vi "GUI_Bella_Control_Center.vi"() -> ()   [LabVIEW 2020]
uses:
  Shared/GUI_Template/GUI_master/tcp_new_data_event.ctl
  Shared/GUI_Template/GUI_master/tcp new data cluster.ctl
  GUI_TestStand/Fire button.ctl
  Device Drivers/DG645/subVIs/TriggerSource_TypDef.ctl
  <vilib>/Utility/config.llb/Write Key (I32).vi
  <vilib>/Platform/browser.llb/Open URL in Default Browser (string).vi
  <vilib>/Utility/config.llb/NI_LVConfig.lvlib
  <vilib>/Utility/config.llb/Read Key (Double).vi
  <vilib>/Utility/config.llb/Write Key (Double).vi
panel:
  in  "delay.Channel_D::32":dbl caption="jet open time D" min=-0.1 max=0.1 format="%.3p"
  in  "delay.Channel_C::32":dbl caption="jet open C" min=-0.1 max=0.1 format="%.3p"
  out "CurrentStatus":string
  in  "MoveStage":bool
  in  "Position.Ch1::44":dbl caption="Current Position" min=0.0 max=150.0
  in  "GUIdevice 44":string="STAGE-LT-Megattenuator"
  in  "GUIdevice 43":string="MANPAR-BELLA-OFI-Boolean"
  in  "GUIdevice 42":string="MANPAR-BELLA-OFI"
  in  "Pressure.device 2::39":dbl caption="Backing pressure" min=-20.0 max=500.0 format="%.3f"
  in  "read config":bool caption="LogTable"
  in  "value5::42":dbl=566.0 caption="2BL probe 0 time pos" min=-9999999.0 max=9999999.0 format="%#_13g"
  in  "save config":bool caption="LogTable"
  in  "configuration file path":path=path "N:/Software/GEECS/user data/BCC.ini"
  out "HPD2 to match HPD":dbl
  in  "Save screenshots":bool
  out "error out":errorcluster
  out "Hpd pos for jet exit":dbl
  in  "value2::42":dbl=276.0 caption="jet exit on hpd for hexX=0" min=-9999999.0 max=9999999.0
  in  "GUIdevice 41":string="STAGE-PL1-JetLength"
  in  "position::41":dbl caption="Jet Length pos" min=0.0 max=50.0 format="%.1f"
  out "lp mode HPDplane\n - HPD ref pos":dbl
  out "height above jet":dbl
  in  "value3::42":dbl=2.6 caption="zpos for 0 above jet" min=-9999999.0 max=9999999.0
  out "HPD - focus":dbl
  in  "value1::42":dbl=230.0 caption="focus on HPD" min=-9999999.0 max=9999999.0
  out "1BL wrt 2BL probe":dbl
  out "1BL delay (ns)\n+ is 1BL after 2BL":dbl
  out "probe delay (ns)\n+ is probe after":dbl caption="probe delay (ns)\n+ is probe after 2BL"
  in  "position::40":dbl caption="2BL probe delay (mm)" min=0.0 max=578.0 format="%.1f"
  in  "GUIdevice 40":string="STAGE-2BL-ProbeDelay"
  in  "Position.Axis 1::8":dbl caption="1BL delay (mm)" min=-500.0 max=500.0 format="%.1f"
  in  "GUIdevice 8":string="STAGE-LT-1BLDelay"
  in  "value4::42":dbl=0.006 caption="JetOnTime" min=-9999999.0 max=9999999.0 format="%#_6p"
  in  "Position.Channel 5::25":dbl caption="SMFiber (1in, 45out)" min=-60.0 max=55.0 format="%.1f"
  in  "value1::43":bool=TRUE caption="GasJetOn"
  in  "value0::43":bool=TRUE caption="ShotControl"
  in  "Thales.DIAG_CU_Output_Percent_1::37":dbl caption="Amp2 att (%)" min=1.0 max=100.0 step=500.0 format="%.2f"
  in  "GUIdevice 37":string="SVE-LT-Thales"
  in  "Pressure.device 1::39":dbl caption="Backing pressure" min=-20.0 max=500.0 format="%.3f"
  in  "GUIdevice 39":string="PRC-PL1-HighPressure"
  in  "Scan":T1(ring)
  in  "LogTable":bool
  in  "New Google\nExpLog for new day?":bool=TRUE
  out "standard output":string
  in  "Create Log":bool caption="LogTable"
  in  "GUIdevice 38":string="STAGE-2BL-Compressor"
  in  "Position.Axis 1::38":dbl caption="Comp2 Translation" min=0.0 max=20.0 format="%.3f"
  in  "Position.Channel 5::31":T2(ring) caption="FROG foil"
  in  "Position.Channel 2::31":T2(ring) caption="Little Rick"
  in  "AnalogOutput.Channel 1::36":dbl caption="M4A att (V)" min=0.0 max=5.0 step=500.0 format="%.2f"
  in  "GUIdevice 36":string="ATT-2BL-M4A"
  in  "GUIdevice 35":string="ATT-2BL-DM"
  in  "AnalogOutput.Channel 1::35":dbl caption="2BL DM att (V)" min=0.0 max=5.0 step=500.0 format="%.2f"
  in  "Step size 2":dbl=20.0 caption="Step size" min=-22.0 max=22.0
  in  "Position.Axis 4::33":dbl caption="Holy M V F4" min=-100000.0 max=100000.0 step=500.0
  in  "Position.Axis 3::33":dbl caption="Holy M H F3" min=-1000000.0 max=1000000.0 step=500.0
  in  "Position.Axis 2::33":dbl caption="Bessel M3 V F2" min=-100000.0 max=100000.0 step=500.0
  in  "Position.Axis 1::33":dbl caption="Bessel M3 H F1" min=-100000.0 max=100000.0 step=500.0
  in  "GUIdevice 33":string="MCD-PL1-picosOFI1"
  in  "delay.Channel_B::32":dbl caption="jet open time B" min=-0.1 max=0.1 format="%.3p"
  in  "delay.Channel_A::32":dbl caption="jet open A" min=-0.1 max=0.1 format="%.3p"
  in  "GUIdevice 32":string="DDG-AA-SRSGasJet-645"
  in  "position::6":dbl caption="LPmode stage long (605 safe)" min=0.0 max=605.0 format="%.1f"
  in  "GUIdevice 6":string="STAGE-PL1-LPmodeLong"
  in  "EnableMotor::6":bool caption="LPmode motor \nstatus"
  in  "position::4":dbl=-1.631e-06 caption="Capstage" min=0.0 max=600.0 format="%.1f"
  in  "GUIdevice 4":string="STAGE-PL1-Capstage1"
  in  "GUIdevice 31":string="1WIRE-BELLA-Flipper"
  in  "Amplitude.Ch GH::10":dbl=-1.631e-06 caption="Shot Shutter V" min=0.5 max=5.0 format="%.1f"
  in  "Rate (Hz)":dbl=0.3
  out "Crystal2":enum16{"In", "Out", "Unknown"}(ring)
  out "Hex1posdesc":enum16{"guiding", "fiber ref", "Unknown"}(ring) caption="Hex1"
  in  "GUIdevice 29":string="MCD-HEAT-ESP0"
  in  "Position.Axis 2::29":dbl caption="Y" min=-5.0 max=25.0 format="%.4f"
  in  "Position.Axis 1::29":dbl caption="X" min=-5.0 max=25.0 format="%.4f"
  in  "wangle::28":dbl caption="w" min=-2.0 max=2.0 step=0.01 format="%.5f"
  in  "vangle::28":dbl caption="v" min=-5.0 max=5.0 step=0.01 format="%.5f"
  in  "uangle::28":dbl caption="u" min=-1.0 max=1.0 step=0.01 format="%.5f"
  in  "ypos::28":dbl caption="y" min=-3.0 max=3.0 step=0.01 format="%.5f"
  in  "zpos::28":dbl caption="z" min=-12.5 max=12.5 step=0.01 format="%.5f"
  in  "xpos::28":dbl caption="x" min=-0.5 max=0.5 step=0.01 format="%.5f"
  in  "GUIdevice 28":string="HEX-PL1-2"
  in  "delay.Channel_A::27":dbl caption="Disch timing both caps" min=-0.1 max=0.1 format="%.3p"
  out "Boolean":bool
  in  "amplitude.Channel_A::27":dbl caption="Caps Trig (V)" min=-3.0 max=4.0 format="%.2f"
  in  "GUIdevice 27":string="DDG-AA-SRS3"
  in  "GUIdevice 26":string="PRC-PL1-PressureAPL"
  in  "pressure::26":dbl caption="Cap2 Pressure (Torr)" min=0.0 max=50.0 format="%.2f"
  in  "Position.Channel 5::25":dbl caption="Wedge (43.5,2)" min=-60.0 max=55.0 format="%.1f"
  in  "Position.Channel 4::25":dbl caption="ND2 (4,45)" min=-35.0 max=-12.0 format="%.1f"
  in  "Position.Channel 1::25":dbl caption="LPmode kicker (~1in, 75out)" min=-75.0 max=79.0 format="%.1f"
  in  "Position.Channel 1::25":dbl caption="ND3 (4,45)" min=-75.0 max=79.0 format="%.1f"
  out "Data.Channel 2::14":dbl caption="Flow US (sccm)" min=0.0 max=1000.0 format="%.1f"
  out "pressure2::5":dbl caption="PDR US (Torr)" min=-100.0 max=500.0 format="%.2f"
  in  "Data.Channel 2::11":dbl caption="Pressure US (Torr)" min=0.0 max=1000.0 format="%.2f"
  in  "GUIdevice 25":string="STAGE-PL1-Smaract"
  in  "Heater Alignment Directions":bool
  in  "Position.Axis 3::15":dbl caption="XY" min=-3.0 max=16.0 format="%.4f"
  in  "Position.Axis 2::15":dbl caption="Y" min=-3.0 max=17.0 format="%.4f"
  in  "Position.Axis 1::15":dbl caption="X" min=-3.0 max=13.0 format="%.4f"
  in  "GUIdevice 24":string="STAGE-HEAT-TL1"
  in  "Encoder position::23":dbl caption="position HPD2" min=0.0 max=600.0 format="%.1f"
  in  "position::3":dbl caption="position HPD" min=0.0 max=600.0 format="%.1f"
  in  "GUIdevice 23":string="STAGE-HPD-Far"
  in  "GUIdevice 22":string="MANPAR-BELLA-FireCont"
  in  "Allow Fire Continues":bool
  out "Fire continues Indicator":bool caption="firing"
  in  "Fire Button":T3=TRUE
  in  "Trigger.Source::10":T4 caption="SRS Trigger Mode"
  out "Absolute Heater timing":dbl caption="delay" format="%#.4p"
  out "Absolute discharge timing":dbl caption="delay from pk" format="%#.3p"
  in  "delay.Channel_A::19":dbl caption="Timing box" min=-0.1 max=0.1 format="%#.4p"
  in  "Delay.Ch E::17":dbl caption="Timing box" min=-0.1 max=0.1 format="%.3p"
  in  "value0::22":bool caption="Fire continuosly"
  in  "voltage::20":dbl caption="Discharge HV (kV)" min=0.0 max=40.0 format="%.2f"
  in  "GUIdevice 20":string="HV-PL1-Glassman"
  in  "SlaveValue::11":dbl caption="Slave Value (%)" min=0.0 max=200.0 format="%.1f"
  in  "GUIdevice 19":string="DDG-HEAT-SRS1"
  in  "GUIdevice 15":string="MCD-HEAT-ESP1"
  in  "GUIdevice 17":string="DDG-AA-SRS0"
  out "error IO 2":errorcluster
  out "fire::10":string
  out "tcp data event":T5
  in  "UDP error message":string
  in  "GUIdevice 14":string="GAUGE-PL1-FlowStage1"
  in  "GUIdevice 13":string="DDG-AA-SRS2"
  in  "GUIdevice 2":string="MANPAR-BELLA-General"
  in  "GUIdevice 10":string="DDG-AA-ShotCntrl"
  in  "GUIdevice 5":string="GAUGE-PL1-Pressure"
  in  "GUIdevice 1":string="HEX-PL1-1"
  in  "GUIdevice 3":string="STAGE-HPD-Tel"
  in  "GUIdevice 11":string="PRC-PL1-Stage1"
  in  "Delay.Ch E::13":dbl caption="Discharge timing (s)" min=-0.1 max=0.2 format="%#_9p"
  in  "<command>::1":bool caption="ABORT\nHEXAPOD"
  in  "Step size":dbl min=-22.0 max=22.0 format="%.5f"
  in  "wangle::1":dbl caption="w (F11 F12)" min=-6.0 max=6.0 step=0.01 format="%.5f"
  in  "vangle::1":dbl caption="v (F9 F10)" min=-6.0 max=6.0 step=0.01 format="%.5f"
  in  "uangle::1":dbl caption="u (F7 F8)" min=-6.0 max=6.0 step=0.01 format="%.5f"
  in  "ypos::1":dbl caption="y (F3 F4)" min=-8.0 max=8.0 step=0.01 format="%.5f"
  in  "zpos::1":dbl caption="z (PgU PgD)" min=-12.0 max=15.0 step=0.01 format="%.5f"
  in  "xpos::1":dbl caption="x (F1 F2)" min=-25.0 max=22.0 step=0.01 format="%.5f"
  in  "Position.Axis 1::9":dbl caption="Comp1 Translation" min=-50.0 max=50.0 format="%.3f"
  in  "GUIdevice 9":string="STAGE-1BL-Compression"
  out "Data.Channel 1::14":dbl caption="Flow DS (sccm)" min=0.0 max=1000.0 format="%.1f"
  in  "Data.Channel 1::11":dbl caption="Pressure DS (Torr)" min=0.0 max=1000.0 format="%.2f"
  out "pressure::5":dbl caption="PDR DS (Torr)" min=-100.0 max=500.0 format="%.2f"
  in  "Delay.Ch C::10":dbl caption="Jet timing (s)" min=-0.1 max=2.1 format="%#_6p"
  in  "stop":bool
  # "BELLA CONTROL CENTER"
  # "CAP"
  # "Hex2"
  # "HEX 1 JET"
  # "HEX 2 Axicon"
  # "PICOS"
  # "DG"
  # "Scan"
  # "Discharge timing (s)"
  # "1wire"
  # "Jet"
  # "Heater timing (s)"
  # "\"-x\" is laser propagation direction"
  # "HPD Stage"
  # "PL1 stages"
  # "Megattenuator Stage"
  # "Attenuate"
  # "OUT"
  # "IN"
  # "Compressors"
  # "needs manpar-bella-ofi on\nMANPAR-BELLA-OFI-Boolean"
  # "Heater Alignment"
  # "Heat ESP0"
  # "Heat ESP1"
  # "Heat Pico"
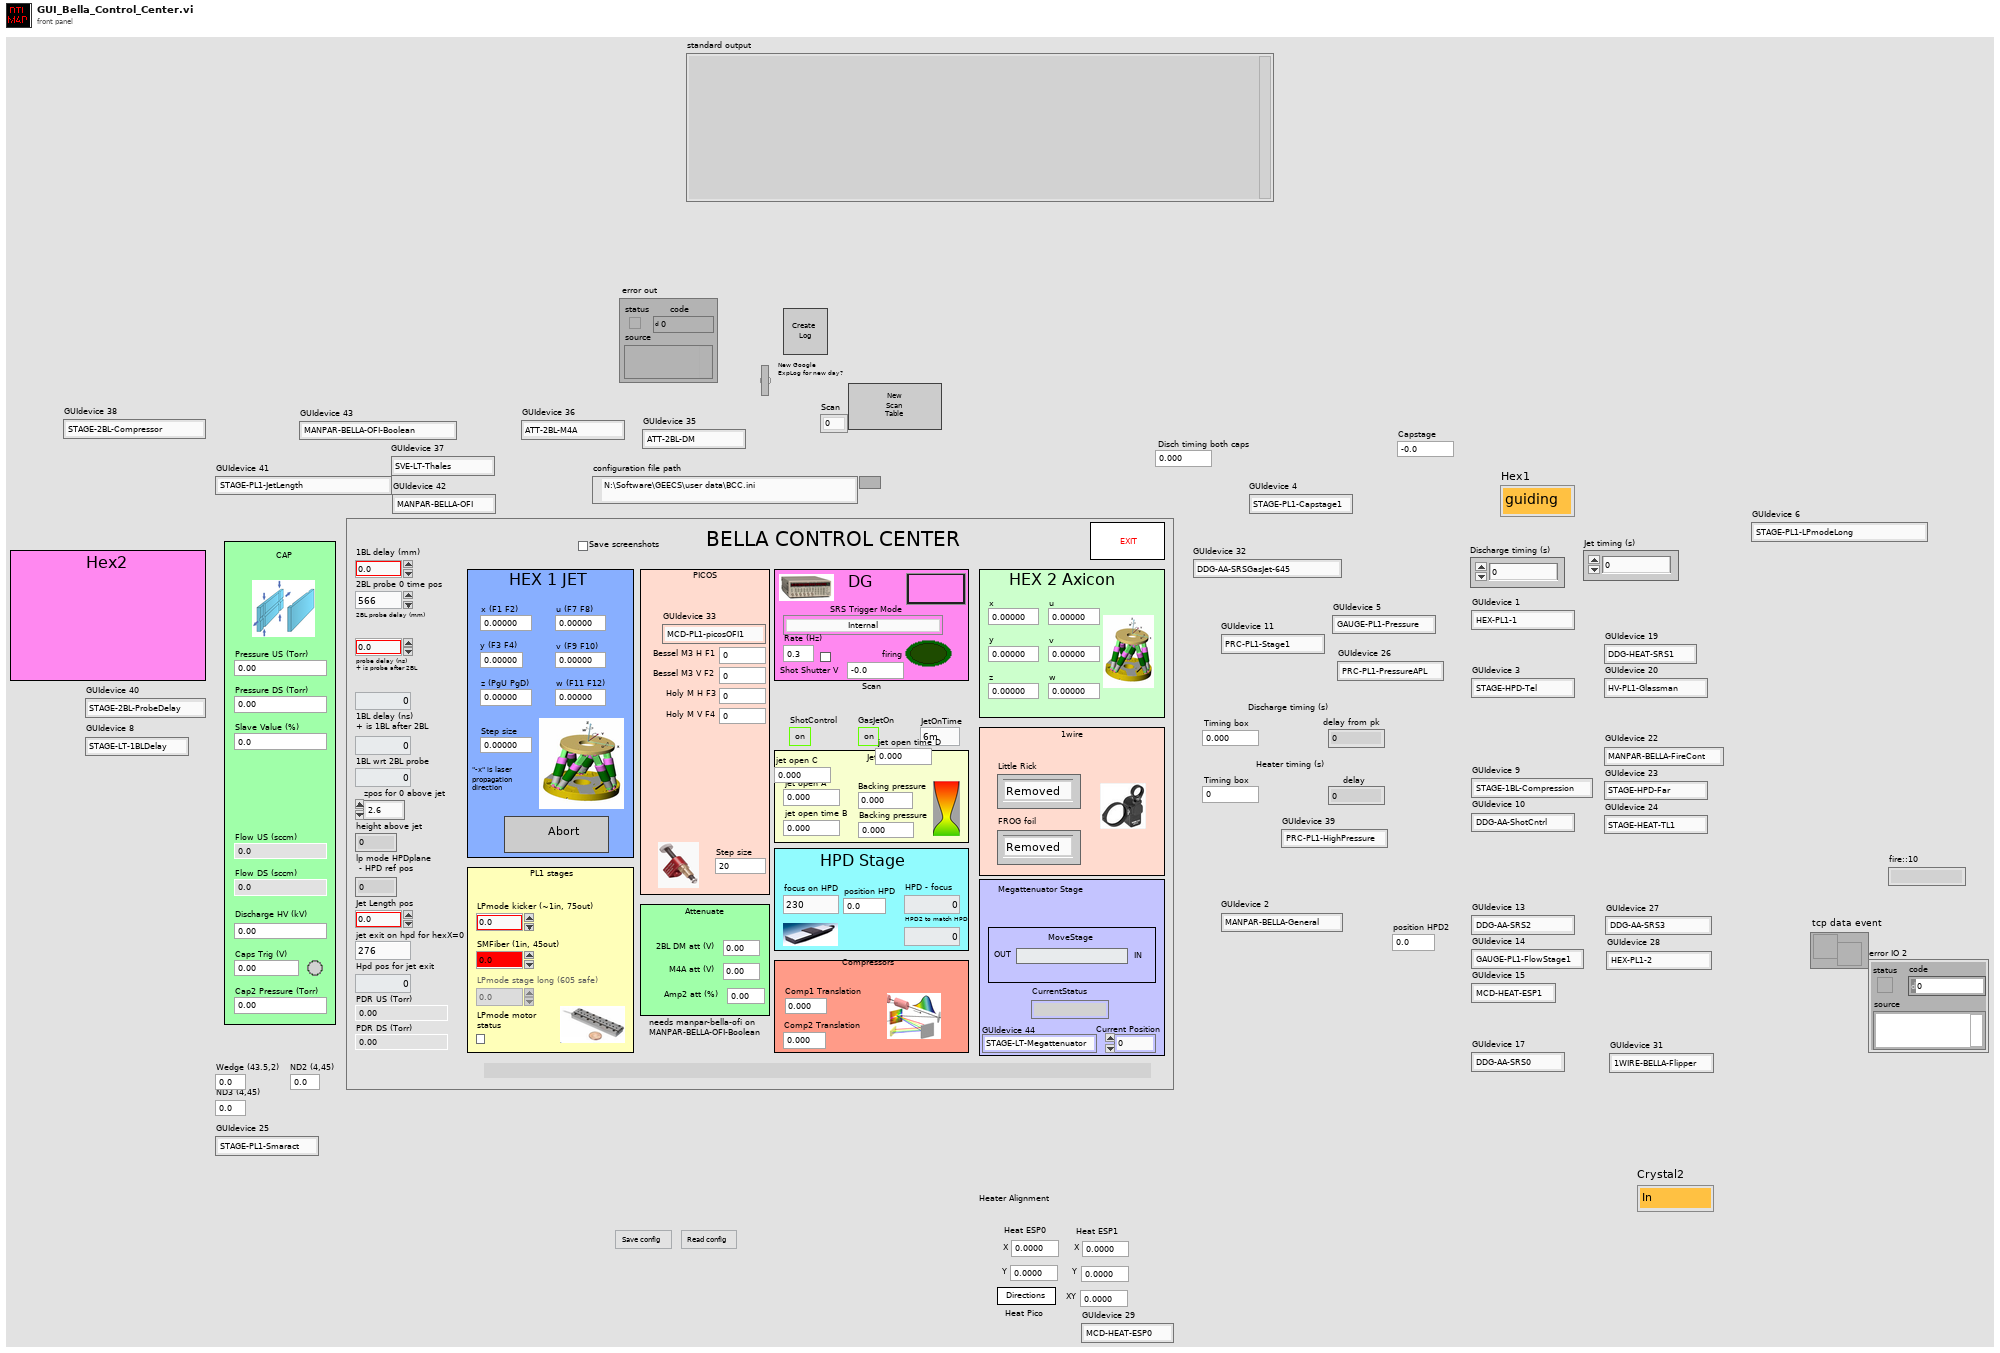
[diagram p1: front panel]
types:
  T1 = enum16{"0", "1", "2", "3", "4", "5", "6", "7", "8", "9", "10", "11", "12", "13", "14", "15", "16", "17", "18", "19", "20", "21", "22", "23", "24", "25", "26", "27", "28", "29", "30", "31", "32", "33", "34", "35", "36", "37", "38", "39", "40", "41", "42", "43", "44", "45", "46", "47", "48", "49", "50", "51", "52", "53", "54", "55", "56", "57", "58", "59", "60", "61", "62", "63", "64", "65", "66", "67", "68", "69", "70", "71", "72", "73", "74", "75", "76", "77", "78", "79", "81", "82", "83", "84", "85", "86", "87", "88", "89", "90", "91", "92", "93", "94", "95", "96", "97", "98", "99", ""}
  T2 = enum16{"Removed", "Inserted", "Unknown", "Moving"}
  T3 = typedef "Fire button.ctl" = bool
  T4 = typedef "TriggerSource_TypDef.ctl" = enum16{"Internal", "External rising edges", "External falling edges", "Single shot external rising edges", "Single shot external falling edges", "Single shot", "Line"}
  T5 = typedef "tcp_new_data_event.ctl" = refnum<user-event>
  T6 = typedef "tcp new data cluster.ctl" = cluster{"EventEnum":enum16{"new data", "connection status update"}, "Device name":string}
  T7 = enum8{"Enabled", "Disabled", "Disabled and Grayed Out"}
  T8 = enum32{"invalid app kind", "Development System", "Run Time System", "Student Edition", "Embedded LabVIEW", "Evaluation", "Custom"}
  T9 = enum32{"Invalid", "Standard", "Closed", "Hidden", "Minimized", "Maximized"}
  T10 = typedef "imagedata.ctl" = cluster{"image type":i32, "image depth":i32, "image":u8[], "mask":u8[], "colors":u32[], "Rectangle":cluster{"left":i16, "top":i16, "right":i16, "bottom":i16}}
  T11 = typedef "NI_LVConfig.lvlib/Config Data RefNum.ctl" = refnum<k1>
  T12 = cluster{"Core":cluster{"Current VI Reference":refnum<vi>, "Close Panel on Exit?":bool}, "Heater timing offset":dbl, "Discharge timing offset":dbl, "Jet trigger":bool, "Tik1":u32, "Tik2":u32, "Fire Continues Allowed":bool, "Config":cluster{"Config Strings":string[], "Config refs":refnum<vi>[]}}
  T13 = cluster{"Config Strings":string[], "Config refs":refnum<vi>[]}
  T14 = cluster{"Current VI Reference":refnum<vi>, "Close Panel on Exit?":bool}
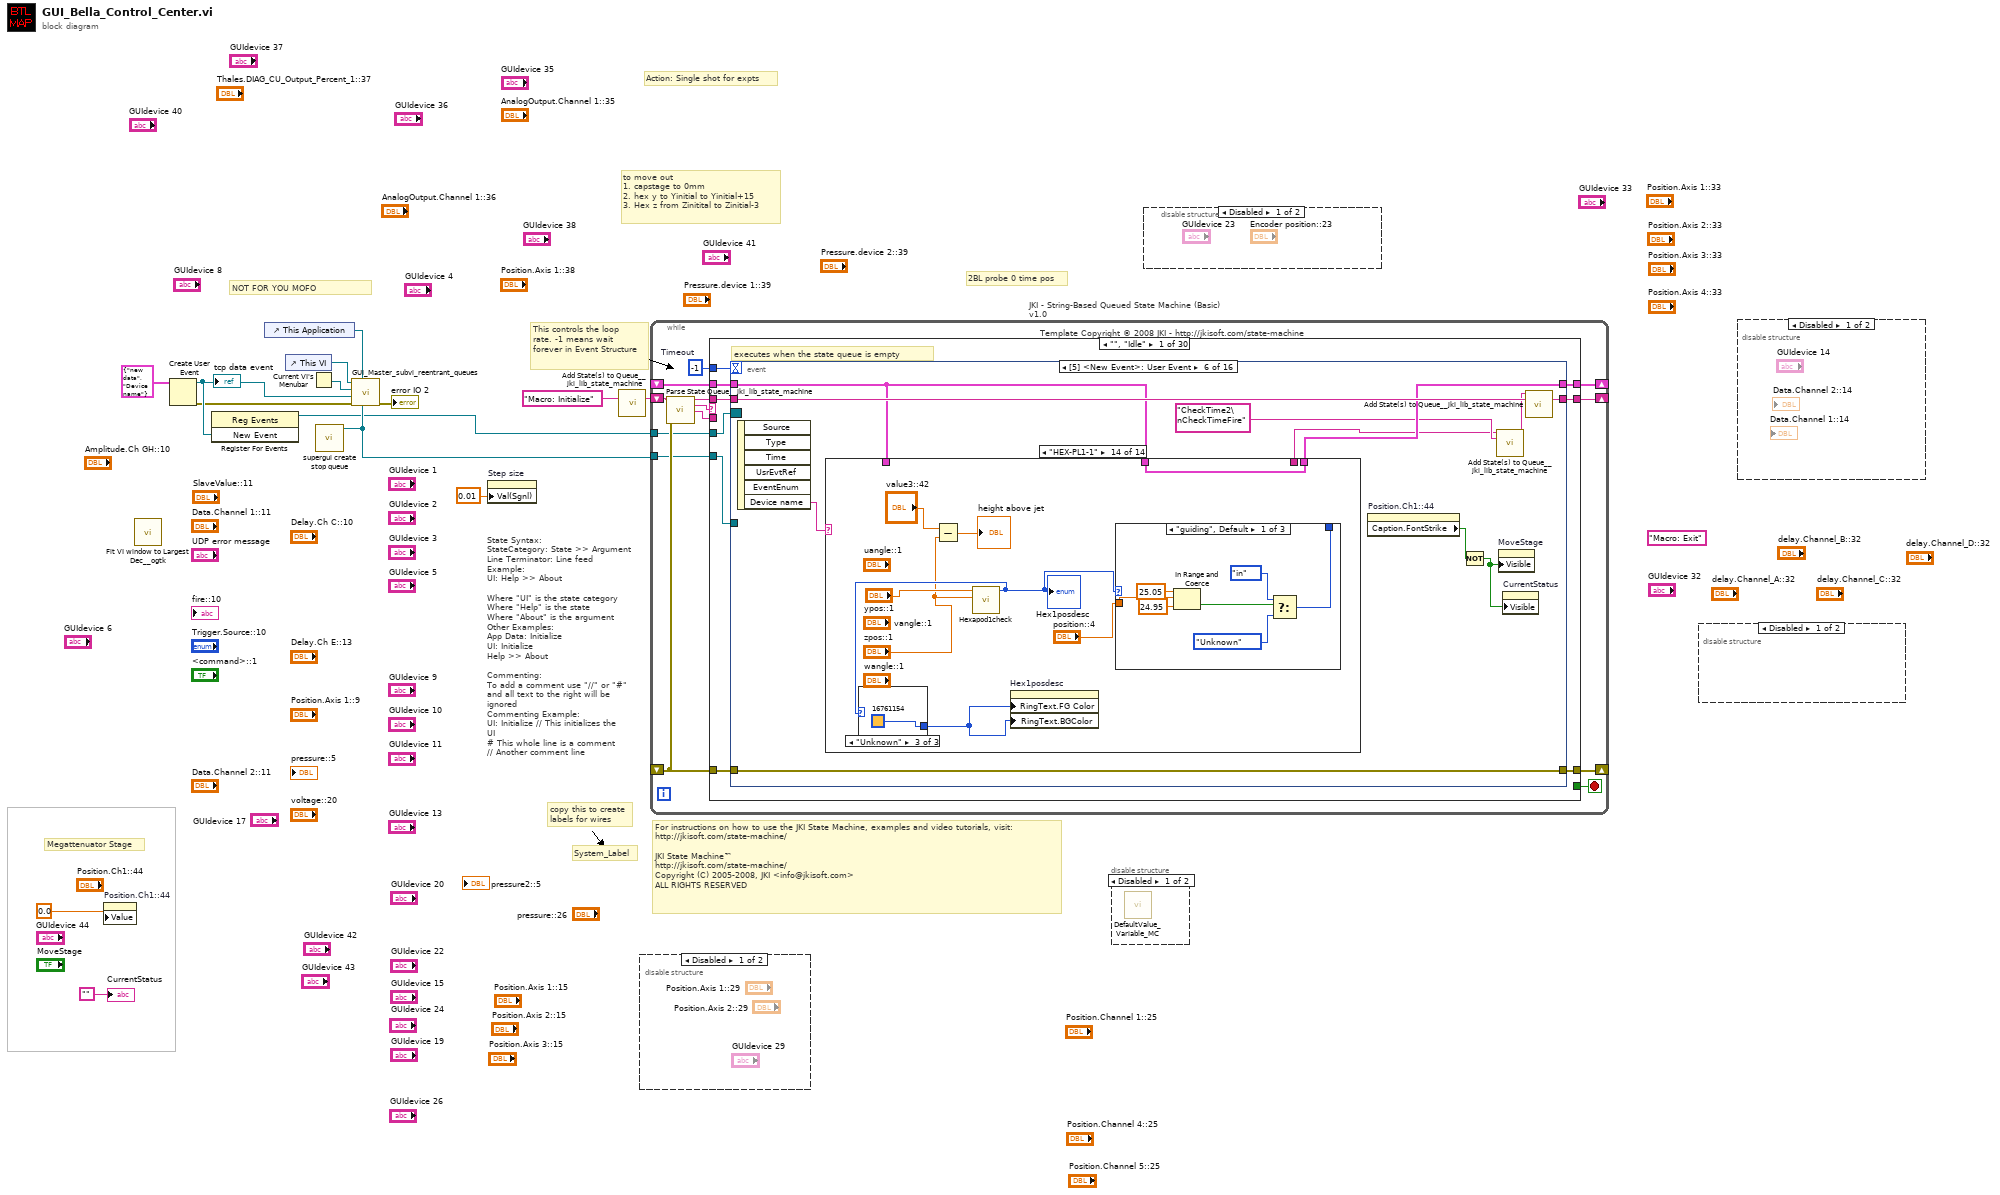
[diagram p0: block diagram]
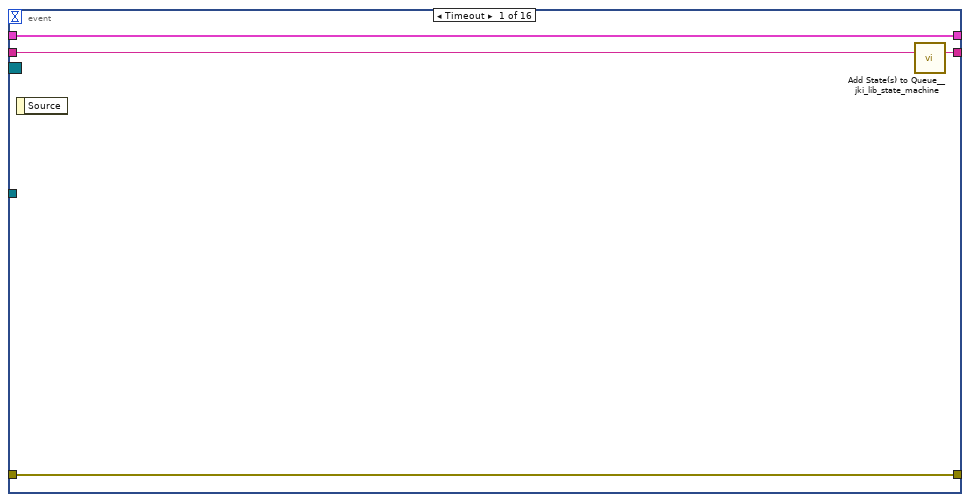
[diagram p7: hidden frame]
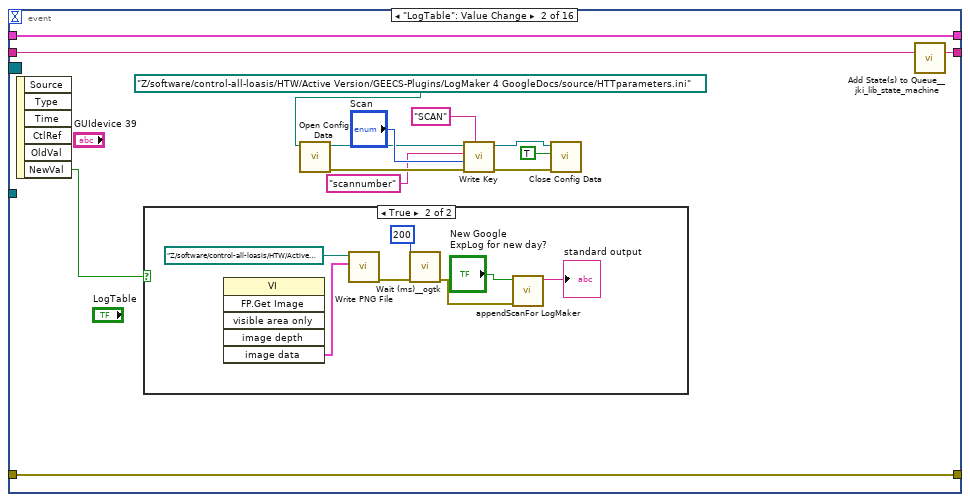
[diagram p8: hidden frame]
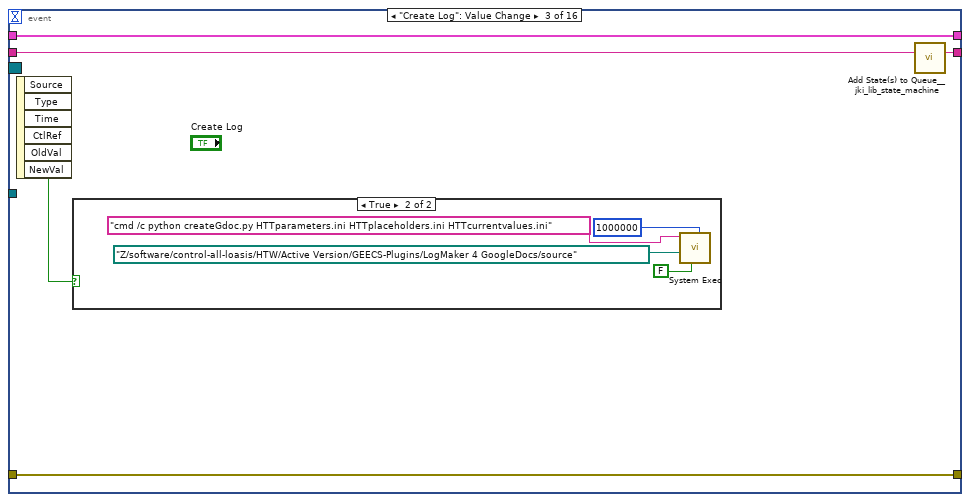
[diagram p10: hidden frame]
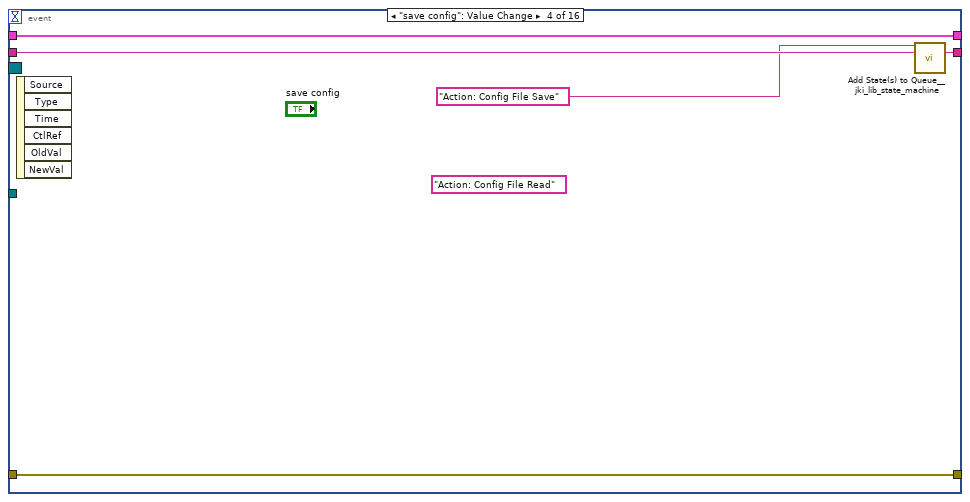
[diagram p12: hidden frame]
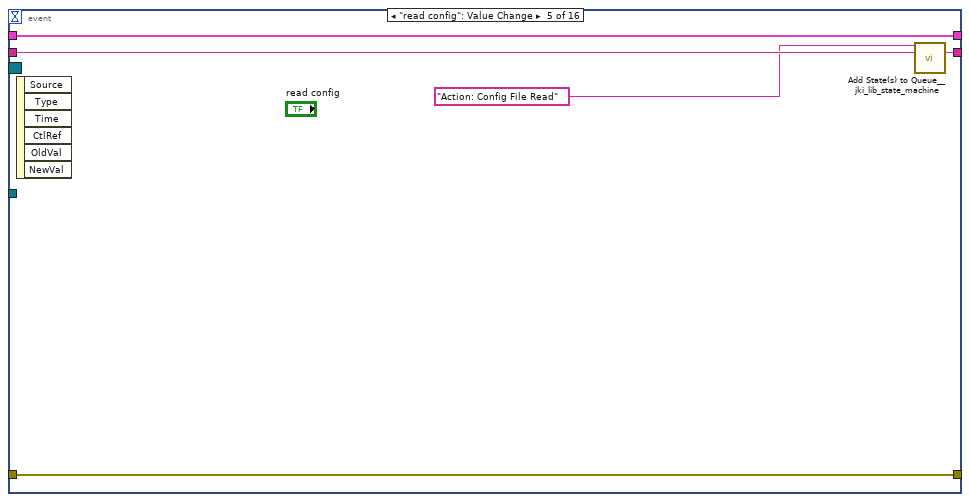
[diagram p13: hidden frame]
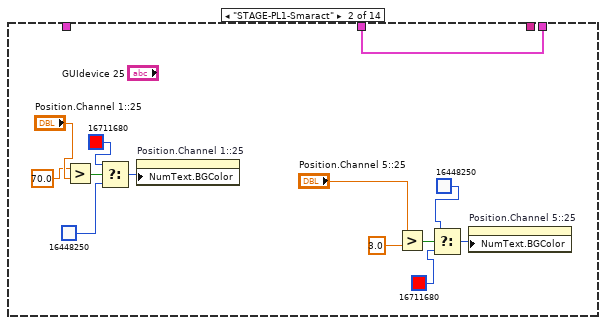
[diagram p15: hidden frame]
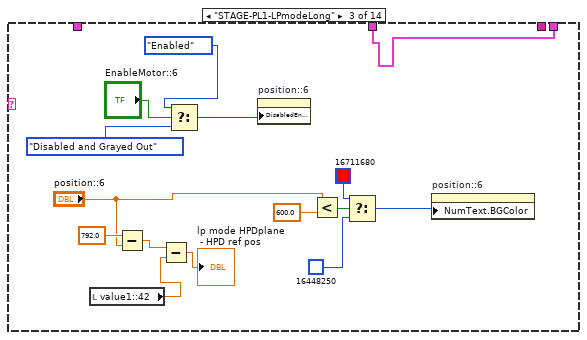
[diagram p16: hidden frame]
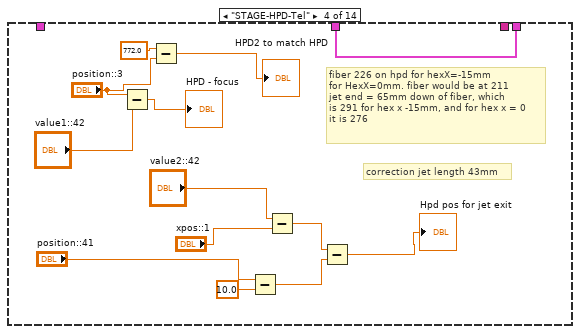
[diagram p17: hidden frame]
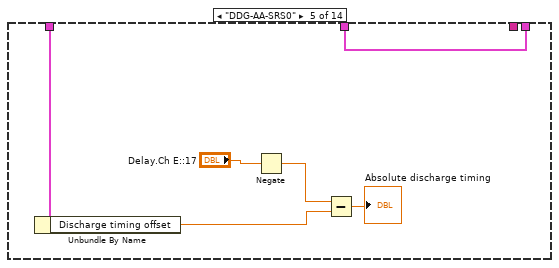
[diagram p18: hidden frame]
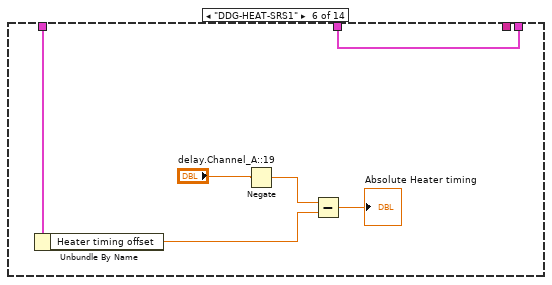
[diagram p19: hidden frame]
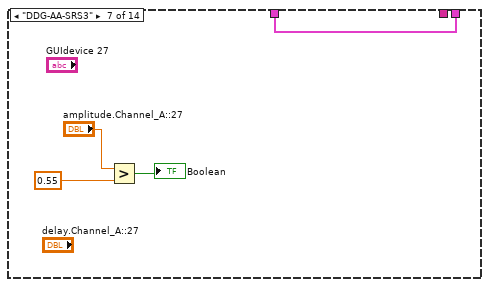
[diagram p20: hidden frame]
diagram:
  (unwired) "Macro: Exit"
  # "Megattenuator Stage"
  # "2BL probe 0 time pos"
  # "Action: Single shot for expts"
  # "to move out\n1. capstage to 0mm\n2. hex y to Yinitial to Yinitial+15\n3. Hex z from Zinitital to Zinitial-3"
  # "For instructions on how to use the JKI State Machine, examples and video tutorials, visit:\nhttp://jkisoft.com/state-machine/\n\nJKI State Machine™\nhttp://jkisoft.com/state-machine/\nCopyright (C) 2005-2008, JKI <info@jkisoft.com>\nALL RIGHTS RESERVED"
  # "State Syntax:\nStateCategory: State >> Argument\nLine Terminator: Line feed\nExample:\nUI: Help >> About\n\nWhere \"UI\" is the state category\nWhere \"Help\" is the state\nWhere \"About\" is the argument\nOther Examples:\nApp Data: Initialize\nUI: Initialize\nHelp >> About\n\nCommenting:\nTo add a comment use \"//\" or \"#\" and all text to the right will be ignored\nCommenting Example:\nUI: Initialize // This initializes the UI\n# This whole line is a comment\n// Another comment line"
  # "copy this to create labels for wires"
  # "This controls the loop rate. -1 means wait forever in Event Structure"
  # "System_Label"
  # "NOT FOR YOU MOFO"
  n1 = property on="Position.Ch1::44" class="DigNum (strict)"("Value"=0.0 ("Position.Ch1::44")) -> ()  [unwired: 2 in, 2 out]
  n2 = call <userlib>:"Fit VI window to Largest Dec__ogtk.vi"() -> ()  [unwired: 6 in, 2 out]
  n3 = Create User Event(user event datatype=T6 {"EventEnum"=enum."new data", "Device name"="Device name"} ("New Event")) -> (user event=w13:refnum<user-event>, error out=w12:errorcluster)  [unwired: 1 in]
  "tcp data event" <- w13
  n4 = register-events(w13) -> (reference out=w3:refnum<event-registration>)  [unwired: 2 in, 1 out]
  n5 = control-ref of="This Application"() -> (w14:refnum<vi>)
  n6 = control-ref of="This VI"() -> (w7:refnum<vi>)
  n7 = Current VI's Menubar() -> (w10:refnum<k9>)
  n8 = call "supergui create stop queue.vi"() -> ("STOP Queue out"=w4:refnum<queue>)  [unwired: 11 in]
  n9 = call "GUI_Master_subvi_reentrant_queues.vi"("STOP Queue in"=w4, "This Application"=w14, "error in (no error)"=w12, "tcp data event"=w13, "Caller menu reference"=w10, "Caller VI ref"=w7) -> ("error out"=→"error IO 2":errorcluster)  [unwired: 5 in]
  n10 = property on="Step size" class="DigNum (strict)"("Val(Sgnl)"=0.01 ("Value (Signaling)")) -> ()  [unwired: 2 in, 2 out]
  n11 = call <vilib>:"Add State(s) to Queue__jki_lib_state_machine.vi"("State(s) in (\"\")"="Macro: Initialize") -> ("States Out"=w5:string)  [unwired: 14 in]
  n12 = disable-structure shown="Disabled" {
    frame Disabled {
    }
    frame Enabled {
    }
  }
  n13 = while "JKI - String-Based Queued State Machine (Basic) v1.0" {
    shift-right: [w20] -> _
    shift-left: _ -> [w19]
    shift-right: [w23] -> _
    shift-left: _ -> [w17]
    shift-right: [w22] -> _
    shift-left: w5 -> [w24]
    tunnel: w3 -> [w16]
    tunnel: w4 -> [w15]
    stop <- w21 stop-if-true
    w18 = -1  # Timeout
    # "Template Copyright © 2008 JKI - http://jkisoft.com/state-machine"
    n14 = call <vilib>:"Parse State Queue__jki_lib_state_machine.vi"("State Queue"=w24, "Error In (no error)"=w17) -> ("Remaining States"=w26:string, "Current State"=w27:string, "Arguments"=w25:string)  [unwired: 11 in]
    n15 = case shown="\"\", \"Idle\"" w27 {
      selector: w27 -> [_ _ w332 _ _ _ _ _ _ _ _ _ _ _ _ _ _ _ _ _ _ _ _ _ _ _ _ _ _ _]
      tunnel: w26 -> [w36 w331 w336 w354 w360 w365 w369 w389 w395 w399 w403 w408 w440 w466 w477 w503 w508 w521 w525 w531 w553 w590 w601 w613 w625 w634 w652 w660 w668 w673]
      tunnel: w25 -> [_ _ _ _ _ _ _ _ _ _ _ _ _ w461 w471 _ _ _ _ w527 _ _ _ _ _ _ w645 _ _ _]
      tunnel: w19 -> [w34 w328 w334 w345 w357 w363 w366 _ w390 w396 w401 w404 w438 w464 w473 w500 w505 w518 w522 w528 w550 w578 w597 w607 w622 w632 w650 w657 w665 w670]
      tunnel: [w33 w329 w338 w351 errorcluster {"status"=FALSE, "code"=0, "source"=""} ("error out") w362 w367 w386 w391 w397 w400 w405 w436 w462 w474 w501 w506 w519 w523 w529 w551 w588 w595 w602 w623 w629 w646 w658 w666 w671] -> w23
      tunnel: w17 -> [w32 w329 w337 w351 w356 w362 w367 w386 w392 w397 w400 w406 w437 w463 w475 w501 w506 w519 w523 w529 w551 w588 w599 w603 w623 w630 w647 w658 w666 w671]
      tunnel: [w35 w330 w335 w353 w359 w364 w368 w388 w394 w398 w402 w407 w439 w465 w476 w502 w507 w520 w524 w530 w552 w589 w600 w612 w624 w633 w651 w659 w667 w672] -> w22
      tunnel: [_ _ _ _ _ TRUE _ _ _ _ _ _ _ _ _ _ _ _ _ _ _ _ _ _ _ _ _ _ _ _] -> w21
      tunnel: [w28 w328 w334 w352 w357 w363 w366 w387 w390 w396 w401 w404 w438 w464 w473 w500 w505 w518 w522 w528 w550 w587 w597 w606 w621 w632 w650 w657 w665 w670] -> w20
      tunnel: w18 -> [w31 _ _ _ _ _ _ _ _ _ _ _ _ _ _ _ _ _ _ _ _ _ _ _ _ _ _ _ _ _]
      tunnel: w16 -> [w30 _ _ _ _ _ _ _ _ _ _ _ _ _ _ _ _ _ _ _ _ _ _ _ _ _ _ _ _ _]
      tunnel: w15 -> [w29 _ _ _ _ _ _ _ _ _ _ _ _ _ _ _ _ w510 _ _ _ _ _ _ _ _ _ _ _ _]
      frame "", "Idle" {
        # "executes when the state queue is empty"
        n16 = event shown="[5] <New Event>: User Event" {
          selector: w30 -> [_ _ _ _ _ _ _ _ _ _ _ _ _ _ _ _]
          dyn-events: _ -> [_ _ _ _ _ _ _ _ _ _ _ _ _ _ _ _]
          timeout: w31 -> [_ _ _ _ _ _ _ _ _ _ _ _ _ _ _ _]
          tunnel: w36 -> [w40 w54 w66 w75 w80 w91 w229 w231 w236 w244 w253 w276 w286 w293 w296 w327]
          tunnel: [w39 w53 w65 w74 w79 w90 w228 w232 w237 w244 w252 w276 w286 w293 w295 w326] -> w35
          tunnel: w34 -> [w37 w51 w63 w72 w77 w87 w226 w234 w239 w243 w255 w277 w287 w292 w303 w324]
          tunnel: [w38 w52 w64 w73 w78 w89 w227 w233 w238 w241 w258 w275 w285 w291 w302 w325] -> w33
          tunnel: w32 -> [w38 w52 w64 w73 w78 w89 w227 w233 w238 w242 w257 w275 w285 w291 w302 w325]
          tunnel: [w37 w51 w63 w72 w77 w86 w226 w234 w239 w243 w256 w277 w287 w292 w303 w324] -> w28
          tunnel: w29 -> [_ _ _ _ _ _ _ _ _ _ _ _ _ _ _ _]
          event Timeout {
            n17 = event-data() -> ()  [unwired: 1 in, 1 out]
            n18 = call <vilib>:"Add State(s) to Queue__jki_lib_state_machine.vi"("State(s) in (\"\")"=w40) -> ("States Out"=w39:string)  [unwired: 14 in]
          }
          event "LogTable": Value Change {
            n19 = event-data() -> ("NewVal"=w41:bool)  [unwired: 1 in, 5 out]
            n20 = case shown="True" w41 {
              frame False {
              }
              frame True {
                n21 = invoke class="VI" method="FP.Get Image"() -> ("image data"=w61:T10)  [unwired: 6 in, 5 out]
                n22 = call <vilib>:"Write PNG File.vi"("image data"=w61, "path to PNG file"=path "Z:/software/control-all-loasis/HTW/Active Version/GEECS-Plugins/LogMaker 4 GoogleDocs/source/frontpanel.png" ("report file path")) -> ("error out"=w56:errorcluster)  [unwired: 8 in, 1 out]
                n23 = call <userlib>:"Wait (ms)__ogtk.vi"("error in (no error)"=w56, "milliseconds to wait"=u32 200 ("millisecond timer value")) -> ("error out"=w55:errorcluster)  [unwired: 8 in, 1 out]
                n24 = call "appendScanFor LogMaker.vi"("error in (no error)"=w55, "New Google\nExpLog for new day?"="New Google\nExpLog for new day?") -> ("standard output"=→"standard output":string)  [unwired: 9 in]
              }
            }
            n25 = call <vilib>:"Open Config Data.vi"("configuration file path"=path "Z:/software/control-all-loasis/HTW/Active Version/GEECS-Plugins/LogMaker 4 GoogleDocs/source/HTTparameters.ini") -> ("error out"=w48:errorcluster, "refnum"=w46:T11)  [unwired: 8 in, 1 out]
            n26 = call-poly <vilib>:"Write Key.vi"("section"="SCAN", "error in (no error)"=w48, "value"="Scan", "key"="scannumber", "refnum"=w46) -> ("error out"=w49:errorcluster, "refnum out"=w47:T11)  [unwired: 4 in, 1 out]
            n27 = call <vilib>:"Close Config Data.vi"("error in (no error)"=w49, "write file if changed (T)"=TRUE, "refnum"=w47) -> ()  [unwired: 7 in, 2 out]
            n28 = call <vilib>:"Add State(s) to Queue__jki_lib_state_machine.vi"("State(s) in (\"\")"=w54) -> ("States Out"=w53:string)  [unwired: 14 in]
          }
          event "Create Log": Value Change {
            n29 = event-data() -> ("NewVal"=w62:bool)  [unwired: 1 in, 5 out]
            n30 = case shown="True" w62 {
              frame False {
              }
              frame True {
                n31 = call <vilib>:"System Exec.vi"("expected output size  (4096)"=u32 1000000, "run minimized? (F)"=FALSE, "working directory"=path "Z:/software/control-all-loasis/HTW/Active Version/GEECS-Plugins/LogMaker 4 GoogleDocs/source", "command line"="cmd /c python createGdoc.py HTTparameters.ini HTTplaceholders.ini HTTcurrentvalues.ini") -> ()  [unwired: 4 in, 4 out]
              }
            }
            n32 = call <vilib>:"Add State(s) to Queue__jki_lib_state_machine.vi"("State(s) in (\"\")"=w66) -> ("States Out"=w65:string)  [unwired: 14 in]
          }
          event "save config": Value Change {
            (unwired) "Action: Config File Read" ("State(s) in Front (\"\")")
            n33 = event-data() -> ()  [unwired: 1 in, 6 out]
            n34 = call <vilib>:"Add State(s) to Queue__jki_lib_state_machine.vi"("State(s) in Front (\"\")"="Action: Config File Save" ("State(s) in Front (\"\")"), "State(s) in (\"\")"=w75) -> ("States Out"=w74:string)  [unwired: 13 in]
          }
          event "read config": Value Change {
            n35 = event-data() -> ()  [unwired: 1 in, 6 out]
            n36 = call <vilib>:"Add State(s) to Queue__jki_lib_state_machine.vi"("State(s) in Front (\"\")"="Action: Config File Read" ("State(s) in Front (\"\")"), "State(s) in (\"\")"=w80) -> ("States Out"=w79:string)  [unwired: 13 in]
          }
          event User Event {
            n37 = event-data() -> ("Device name"=w88:string)  [unwired: 1 in, 5 out]
            n38 = case shown="\"HEX-PL1-1\"" w88 {
              tunnel: w87 -> [_ _ _ _ w136 w142 _ _ _ _ _ _ _ _]
              tunnel: w87 -> [w92 w105 w120 w133 w134 w140 w148 w153 w163 w167 w175 w182 w184 w207]
              tunnel: [w92 w105 w120 w133 w134 w140 w148 w153 w163 w167 w175 w182 w184 w207] -> w86
              tunnel: [_ _ _ _ _ _ _ _ w162 w166 _ _ _ _] -> w83
              frame "False", Default {
              }
              frame "STAGE-PL1-Smaract" {
                n39 = Greater?(x=70.0 ("y"), y="Position.Channel 1::25") -> (0:w104:bool)
                n40 = Select(t=u32 16711680, s=w104, f=u32 16448250) -> (s? t:f=w101:u32)
                n41 = property on="Position.Channel 1::25" class="DigNum (strict)"("NumText.BGColor"=w101) -> ()  [unwired: 2 in, 2 out]
                n42 = Greater?(x="Position.Channel 5::25", y=3.0) -> (0:w97:bool)
                n43 = Select(t=u32 16448250, s=w97, f=u32 16711680) -> (s? t:f=w100:u32)
                n44 = property on="Position.Channel 5::25" class="DigNum (strict)"("NumText.BGColor"=w100) -> ()  [unwired: 2 in, 2 out]
              }
              frame "STAGE-PL1-LPmodeLong" {
                n45 = local read "value1::42"() -> (w107:dbl)
                n46 = Subtract(x=792.0, y="position::6") -> (x-y=w108:dbl)
                n47 = Subtract(x=w108, y=w107) -> (x-y=→"lp mode HPDplane\n - HPD ref pos":dbl)
                n48 = Select(t=T7."Enabled" ("Disabled"), s="EnableMotor::6", f=T7."Disabled and Grayed Out" ("Disabled")) -> (s? t:f=w111:T7)
                n49 = property on="position::6" class="DigNum (strict)"("DisabledEnum"=w111) -> ()  [unwired: 2 in, 2 out]
                n50 = Less?(x="position::6", y=600.0) -> (x < y?=w119:bool)
                n51 = Select(t=u32 16711680, s=w119, f=u32 16448250) -> (s? t:f=w115:u32)
                n52 = property on="position::6" class="DigNum (strict)"("NumText.BGColor"=w115) -> ()  [unwired: 2 in, 2 out]
              }
              frame "STAGE-HPD-Tel" {
                # "correction jet length 43mm"
                # "fiber 226 on hpd for hexX=-15mm\nfor HexX=0mm. fiber would be at 211\njet end = 65mm down of fiber, which\nis 291 for hex x -15mm, and for hex x = 0\nit is 276"
                n53 = Subtract(x="position::3", y="value1::42") -> (x-y=→"HPD - focus":dbl)
                n54 = Subtract(x=772.0 ("y"), y="position::3") -> (x-y=→"HPD2 to match HPD":dbl)
                n55 = Subtract(x="position::41", y=10.0) -> (x-y=w125:dbl)
                n56 = Subtract(x="value2::42", y="xpos::1") -> (x-y=w126:dbl)
                n57 = Subtract(x=w126, y=w125) -> (x-y=→"Hpd pos for jet exit":dbl)
              }
              frame "DDG-AA-SRS0" {
                n58 = Unbundle By Name(w136) -> ("Discharge timing offset"=w135:dbl)
                n59 = Negate(x="Delay.Ch E::17") -> (-x=w137:dbl)
                n60 = Subtract(x=w137, y=w135) -> (x-y=→"Absolute discharge timing":dbl)
              }
              frame "DDG-HEAT-SRS1" {
                n61 = Unbundle By Name(w142) -> ("Heater timing offset"=w141:dbl)
                n62 = Negate(x="delay.Channel_A::19") -> (-x=w143:dbl)
                n63 = Subtract(x=w143, y=w141) -> (x-y=→"Absolute Heater timing":dbl)
              }
              frame "DDG-AA-SRS3" {
                n64 = Greater?(x="amplitude.Channel_A::27", y=0.55) -> (0:→"Boolean":bool)
              }
              frame "STAGE-2BL-ProbeDelay" {
                n65 = Subtract(x="position::40", y="value5::42") -> (x-y=w158:dbl)
                n66 = Negate(x=w158) -> (-x=w157:dbl)
                n67 = Multiply(x=4.0, y=w157) -> (x*y=w155:dbl)
                n68 = Divide(x=w155, y=299792458000.0) -> (x/y=w152:dbl)
                n69 = Multiply(x=1000000000.0, y=w152) -> (x*y=→"probe delay (ns)\n+ is probe after":dbl)
              }
              frame "MANPAR-BELLA-OFI" {
                n70 = First Call?() -> (First Call?: T/F=w161:bool)
                n71 = case shown="True" w161 {
                  tunnel: [_ "Action: SendScanParameters" ("State(s) in Front (\"\")")] -> w162
                  frame False {
                  }
                  frame True {
                  }
                }
              }
              frame "MANPAR-BELLA-OFI-Boolean" {
                n72 = First Call?() -> (First Call?: T/F=w165:bool)
                n73 = case shown="True" w165 {
                  tunnel: [_ "Action: SendScanParameters" ("State(s) in Front (\"\")")] -> w166
                  frame False {
                  }
                  frame True {
                  }
                }
              }
              frame "STAGE-LT-1BLDelay" {
                n74 = local read "probe delay (ns)\n+ is probe after"() -> (w169:dbl)
                n75 = Subtract(x="Position.Axis 1::8", y=929.0) -> (x-y=w180:dbl)
                n76 = Negate(x=w180) -> (-x=w179:dbl)
                n77 = Multiply(x=2.0, y=w179) -> (x*y=w177:dbl)
                n78 = Divide(x=w177, y=299792458000.0) -> (x/y=w174:dbl)
                n79 = Multiply(x=1000000000.0, y=w174) -> (x*y=w170:dbl)
                "1BL delay (ns)\n+ is 1BL after 2BL" <- w170
                n80 = Subtract(x=w170, y=w169) -> (x-y=→"1BL wrt 2BL probe":dbl)
              }
              frame "1WIRE-BELLA-Flipper" {
              }
              frame "HEX-PL1-2" {
                n81 = disable-structure shown="Disabled" {
                  disable-tunnel: "ypos::28" -> [w188 _]
                  frame Disabled {
                    n82 = Equal?(x=w188, y=15.6) -> (x = y?=w186:bool)
                    n83 = Equal?(x=-20.0 ("y"), y=w188) -> (x = y?=w190:bool)
                    n84 = case shown="False" w190 {
                      tunnel: [w194 enum16{"In", "Out"}."Out" ("sdfsdfs 2")] -> w185
                      tunnel: [w192 u32 16185078] -> w189
                      tunnel: w186 -> [w193 _]
                      frame False {
                        n85 = case shown="False" w193 {
                          tunnel: [enum16{"In", "Out", "Unknown"}."Unknown" ("sdfsdfs 2") enum16{"In", "Out"}."In" ("sdfsdfs 2")] -> w194
                          tunnel: [u32 16761154 ("Color Box") u32 16711680] -> w192
                          frame False {
                          }
                          frame True {
                          }
                        }
                      }
                      frame True {
                      }
                    }
                    "Crystal2" <- w185
                    n86 = property on="Crystal2" class="Enum (strict)"("RingText.FG Color"=w189, "RingText.BGColor"=w189) -> ()  [unwired: 2 in, 2 out]
                  }
                  frame Enabled {
                  }
                }
              }
              frame "HEX-PL1-1" {
                n87 = Subtract(x="value3::42", y="zpos::1") -> (x-y=→"height above jet":dbl)
                n88 = call "Hexapod1check.vi"("zpos::1"="zpos::1", "ypos::1"="ypos::1") -> ("sdfsdfs"=w205:enum16{"guiding", "fiber ref", "Unknown"})  [unwired: 9 in]
                "Hex1posdesc" <- w205
                n89 = case shown="\"Unknown\"" w205 {
                  tunnel: [u32 16448250 u32 16711680 u32 16761154] -> w206
                  frame "guiding", Default {
                  }
                  frame "fiber ref" {
                  }
                  frame "Unknown" {
                  }
                }
                n90 = property on="Hex1posdesc" class="Enum (strict)"("RingText.FG Color"=w206, "RingText.BGColor"=w206) -> ()  [unwired: 2 in, 2 out]
                n91 = case shown="\"guiding\", Default" w205 {
                  tunnel: [w213 w217 enum16{"out", "in", "Unknown"}."Unknown" ("CapStatus")] -> _
                  tunnel: "position::4" -> [w212 w220 _]
                  frame "guiding", Default {
                    n92 = In Range and Coerce(upper limit=25.05, x=w212, lower limit=24.95) -> (In Range?=w209:bool)  [unwired: 1 out]
                    n93 = Select(t=enum16{"out", "in", "Unknown"}."in" ("CapStatus"), s=w209, f=enum16{"out", "in", "Unknown"}."Unknown" ("CapStatus")) -> (s? t:f=w213:enum16{"out", "in", "Unknown"})
                  }
                  frame "fiber ref" {
                    n94 = Equal To 0?(x=w220) -> (x = 0?=w219:bool)
                    n95 = Select(t=enum16{"out", "in", "Unknown"}."out" ("CapStatus"), s=w219, f=enum16{"out", "in", "Unknown"}."Unknown" ("CapStatus")) -> (s? t:f=w217:enum16{"out", "in", "Unknown"})
                  }
                  frame "Unknown" {
                  }
                }
              }
            }
            n96 = property on="Position.Ch1::44" class="DigNum (strict)"() -> ("Caption.FontStrike"=w82:bool)  [unwired: 2 in, 2 out]
            n97 = Not(x=w82) -> (.not. x?=w81:bool)
            n98 = call <vilib>:"Add State(s) to Queue__jki_lib_state_machine.vi"("State(s) in Front (\"\")"=w83, "State(s) in (\"\")"="CheckTime2\nCheckTimeFire" ("State(s) in Front (\"\")")) -> ("States Out"=w84:string)  [unwired: 13 in]
            n99 = property on="MoveStage" class="Bool (strict)"("Visible"=w81) -> ()  [unwired: 2 in, 2 out]
            n100 = property on="CurrentStatus" class="Str"("Visible"=w81) -> ()  [unwired: 2 in, 2 out]
            n101 = call <vilib>:"Add State(s) to Queue__jki_lib_state_machine.vi"("State(s) in Front (\"\")"=w84, "State(s) in (\"\")"=w91) -> ("States Out"=w90:string)  [unwired: 13 in]
          }
          event "stop": Value Change {
            # "Exit Button Value Change (pressed) Event\n(this executes Macro: Exit to terminate the VI)"
            n102 = event-data() -> ()  [unwired: 1 in, 6 out]
            n103 = call <vilib>:"Add State(s) to Queue__jki_lib_state_machine.vi"("State(s) in Front (\"\")"="Macro: Exit", "State(s) in (\"\")"=w229) -> ("States Out"=w228:string)  [unwired: 13 in]
          }
          event Value Change {
            n104 = event-data() -> ()  [unwired: 1 in, 6 out]
            n105 = call <vilib>:"Add State(s) to Queue__jki_lib_state_machine.vi"("State(s) in Front (\"\")"="Action: Fire" ("State(s) in Front (\"\")"), "State(s) in (\"\")"=w231) -> ("States Out"=w232:string)  [unwired: 13 in]
          }
          event "value0::43", "value1::43", "value4::42": Value Change {
            n106 = event-data() -> ()  [unwired: 1 in, 6 out]
            n107 = call <vilib>:"Add State(s) to Queue__jki_lib_state_machine.vi"("State(s) in Front (\"\")"="Action: SendScanParameters" ("State(s) in Front (\"\")"), "State(s) in (\"\")"=w236) -> ("States Out"=w237:string)  [unwired: 13 in]
          }
          event "Heater Alignment Directions": Value Change {
            n108 = event-data() -> ()  [unwired: 1 in, 6 out]
            n109 = case shown="True" "Heater Alignment Directions" {
              tunnel: w242 -> [w245 w248]
              tunnel: [w245 w247] -> w241
              frame False {
              }
              frame True {
                n110 = call-poly <vilib>:"Open URL in Default Browser.vi"("error in (no error)"=w248, "URL"="https://docs.google.com/document/d/1RMZp6W8Kkog2nkTymSjyZ2bh9D7Vo4bxhvGgn3Ut4KE/edit") -> ("error out"=w247:errorcluster)  [unwired: 4 in, 1 out]
              }
            }
          }
          event "Allow Fire Continues": Value Change {
            n111 = event-data() -> ()  [unwired: 1 in, 6 out]
            n112 = Unbundle By Name(w255) -> ("Fire Continues Allowed"=w254:bool)
            n113 = case shown="True" "Allow Fire Continues" {
              tunnel: [w259 w266] -> w258
              tunnel: "Allow Fire Continues" -> [_ w265]
              tunnel: w257 -> [w259 w264]
              tunnel: w254 -> [w260 w263]
              tunnel: [w260 w261] -> w250
              tunnel: [_ "Initilize Fire Continues" ("State(s) in Front (\"\")")] -> w249
              frame False {
              }
              frame True {
                n114 = case shown="False" w263 {
                  tunnel: [w272 w273] -> w266
                  tunnel: w265 -> [w271 _]
                  tunnel: w264 -> [w270 w273]
                  tunnel: [w267 FALSE] -> w261
                  frame False {
                    n115 = call "Password"("Enable"=w271, "error in (no error)"=w270) -> ("Password"=w269:string, "error out"=w272:errorcluster)  [unwired: 15 in, 1 out]
                    n116 = Equal?(x=w269, y="fire") -> (x = y?=w267:bool)
                  }
                  frame True {
                  }
                }
              }
            }
            n117 = Bundle By Name(cluster=w255, "Fire Continues Allowed"=w250) -> (w256:T12)
            n118 = call <vilib>:"Add State(s) to Queue__jki_lib_state_machine.vi"("State(s) in Front (\"\")"=w249, "State(s) in (\"\")"=w253) -> ("States Out"=w252:string)  [unwired: 13 in]
          }
          event "Step size": Value Change {
            n119 = event-data() -> ("NewVal"=w278:dbl)  [unwired: 1 in, 5 out]
            n120 = property on="uangle::1" class="DigNum (strict)"("Increment"=w278) -> ()  [unwired: 2 in, 2 out]
            n121 = property on="vangle::1" class="DigNum (strict)"("Increment"=w278) -> ()  [unwired: 2 in, 2 out]
            n122 = property on="xpos::1" class="DigNum (strict)"("Increment"=w278) -> ()  [unwired: 2 in, 2 out]
            n123 = property on="zpos::1" class="DigNum (strict)"("Increment"=w278) -> ()  [unwired: 2 in, 2 out]
            n124 = property on="wangle::1" class="DigNum (strict)"("Increment"=w278) -> ()  [unwired: 2 in, 2 out]
            n125 = property on="ypos::1" class="DigNum (strict)"("Increment"=w278) -> ()  [unwired: 2 in, 2 out]
          }
          event "Step size 2": Value Change {
            n126 = event-data() -> ("NewVal"=w279:dbl)  [unwired: 1 in, 5 out]
            n127 = control-ref of="Position.Axis 1::33"() -> (w284:refnum<vi>)
            n128 = control-ref of="Position.Axis 2::33"() -> (w283:refnum<vi>)
            n129 = control-ref of="Position.Axis 4::33"() -> (w281:refnum<vi>)
            n130 = control-ref of="Position.Axis 3::33"() -> (w282:refnum<vi>)
            n131 = Build Array(w284, w283, w282, w281) -> (w280:refnum<vi>[])
            n132 = for {
              tunnel: w280 -> [w289] mode=indexing
              tunnel: w279 -> [w288]
              n133 = property on="Property Node" class="DigNum (strict)"(reference=w289, "Increment"=w288) -> ()  [unwired: 1 in, 2 out]
            }
          }
          event Value Change {
            n134 = event-data() -> ()  [unwired: 1 in, 6 out]
            n135 = property on="value0::22" class="Bool (strict)"("Val(Sgnl)"=FALSE) -> ()  [unwired: 2 in, 2 out]
          }
          event "MoveStage": Value Change {
            n136 = event-data() -> ("OldVal"=w298:bool, "NewVal"=w301:bool)  [unwired: 1 in, 4 out]
            n137 = flat-sequence {
              tunnel: w301 -> [w308]
              tunnel: [w308] -> w300
              tunnel: [w305] -> w299
              tunnel: w298 -> [w304]
              tunnel: [w304] -> w297
              tunnel: w300 -> [w312]
              tunnel: w299 -> [w311]
              tunnel: w297 -> [w310]
              tunnel: [w309] -> w294
              frame #0 {
                n138 = call "PasswordPrompt.vi"() -> ("Please enter password below 2"=w307:string)  [unwired: 11 in]
                n139 = Equal?(x=w307, y="l0dat&srv!") -> (x = y?=w305:bool)
              }
              frame #1 {
                n140 = case shown="True" w311 {
                  tunnel: w312 -> [_ w317]
                  tunnel: w310 -> [w314 _]
                  tunnel: ["" w316] -> w309
                  frame False {
                    n141 = call "Display Message to User"("Message"="Wrong Password") -> ()  [unwired: 9 in, 2 out]
                    n142 = property on="MoveStage" class="Bool (strict)"("Value"=w314) -> ()  [unwired: 2 in, 2 out]
                  }
                  frame True {
                    n143 = case shown="False" w317 {
                      tunnel: [" Check Megattenuator Stage Status>>OUT" " Check Megattenuator Stage Status>>IN"] -> w316
                      frame False {
                        n144 = property on="Position.Ch1::44" class="DigNum (strict)"("Val(Sgnl)"=150.0 ("Value (Signaling)")) -> ()  [unwired: 2 in, 2 out]
                      }
                      frame True {
                        n145 = property on="Position.Ch1::44" class="DigNum (strict)"("Val(Sgnl)"=0.5 ("Value (Signaling)")) -> ()  [unwired: 2 in, 2 out]
                      }
                    }
                    n146 = property on="MoveStage" class="Bool (strict)"("Value"=w317) -> ()  [unwired: 2 in, 2 out]
                  }
                }
              }
            }
            n147 = call <vilib>:"Add State(s) to Queue__jki_lib_state_machine.vi"("State(s) in Front (\"\")"=w294, "State(s) in (\"\")"=w296) -> ("States Out"=w295:string)  [unwired: 13 in]
          }
          event Panel Close? {
            # "Discard the event because we'll close the front panel ourselves in Macro: Exit"
            # "Close Panel button (pressed) Event\n(this executes Macro: Exit to terminate the VI)"
            n148 = event-data() -> ()  [unwired: 1 in, 1 out]
            n149 = event-data("Discard?"=TRUE) -> ()  [unwired: 1 in, 1 out]
            n150 = call <vilib>:"Add State(s) to Queue__jki_lib_state_machine.vi"("State(s) in Front (\"\")"="Macro: Exit", "State(s) in (\"\")"=w327) -> ("States Out"=w326:string)  [unwired: 13 in]
          }
        }
      }
      frame "---------- Core ----------" {
        # "Do not put any code in this frame.\n(it is a separator no-op)"
        n151 = call <vilib>:"Add State(s) to Queue__jki_lib_state_machine.vi"("State(s) in (\"\")"=w331) -> ("States Out"=w330:string)  [unwired: 14 in]
      }
      frame Default {
        w341 = 42 items=["No error", "Argument error", "Memory is full", "Out of zone", "End of file", "File already open", "Generic file I/O error", "File not found", "File permission error", "Disk is full", "Duplicate path", "Too many files open", "System feature not enabled", "Resource file not found", "Cannot add resource", "Resource not found", "Image not found", "Image memory error", "Pen does not exist", "Config type invalid", "Config token not found", "Config parse error", "Config memory error", "Bad external code format", "Bad external code offset", "External code not present", "Null window", "Destroy window error", "Null menu", "Print aborted", "Bad print record", "Print driver error", "Windows error during printing", "Memory error during printing", "Print dialog error", "Generic print error", "Invalid device refnum", "Device not found", "Device parameter error", "Device unit error", "Cannot open device", "Device call aborted", "Generic error", "Cancelled by user", "Object ID too low", "Object ID too high", "Object not in heap", "Unknown heap", "Unknown object (invalid DefProc)", "Unknown object (DefProc not in table)", "Message out of range", "Invalid (null) method", "Unknown message", "Manager call not supported", "Bad address", "Network operation in progress", "Network operation timed out", "Connection is busy", "Network attribute not supported", "Network error", "Address in use", "System out of memory", "Connection aborted", "Connection refused", "Not connected", "Already connected", "Connection closed", "Initialization error (interapplication manager)", "Bad occurrence", "Wait on unbound occurrence handler", "Occurrence queue overflow", "Datalog type conflict", "Unused", "Unrecognized type (interapplication manager)", "Memory corrupt", "Failed to make temporary DLL", "Old CIN version", "Drag socket not found", "Failed to load drop-object", "Failed to register OLE object", "Failed to release OLE object", "Format specifier type mismatch", "Unknown format specifier", "Too few format specifiers", "Too many format specifiers", "Scan failed", "Newer CIN version", "Error converting to variant", "Runtime menu error", "Password tampered", "Variant attribute not found", "Incompatible variant data type", "Event data is not available", "Event Store is not present", "Occurrence is not found", "Event Queue is not created", "Event info is not available", "Refnum passed is NULL", "Error retrieving Class GUID", "Error retrieving CoClass GUID", "Error retrieving TypeLib GUID.", "Bad built application magic bytes.", "Specific driver is different from the specific driver associated with the Logical Name.", "There is no session opened to the class driver.", "Max Error", "MAX - Error with config objects", "MAX - Error loading configuration", "MAX - Group not supported"]
        # "Current State"
        # "Do not delete, rename, or modify this frame.\n(this is used to capture unhandled states and typos)"
        # "Handle mistyped state name (developer tool)"
        n152 = Format Into String(format string="Software Exception: Unhandled State \"%s\"." ("message"), error in=w337, w332) -> (resulting string=w340:string, error out=w339:errorcluster)  [unwired: 1 in]
        n153 = call <vilib>:"Error Cluster From Error Code.vi"("show call chain? (False)"=TRUE, "error in (no error)"=w339, "error message (\"\")"=w340, "error code (0)"=w341) -> ("error out"=w338:errorcluster)  [unwired: 5 in]
        n154 = call <vilib>:"Add State(s) to Queue__jki_lib_state_machine.vi"("State(s) in (\"\")"=w336) -> ("States Out"=w335:string)  [unwired: 14 in]
      }
      frame "Initialize Core Data" {
        # "Do not delete, rename, or modify this frame.\n(this is used to determine panel behavior on exit)"
        # "originally closed?"
        # "exe?"
        # "If panel starts closed or is an EXE, then close it when we exit"
        n155 = property class="VI"() -> ("Front Panel.Open"=w350:bool)  [unwired: 2 in, 2 out]
        n156 = property class="App"() -> ("App.Kind"=w349:T8)  [unwired: 2 in, 2 out]
        n157 = control-ref of="Current VI Reference"() -> (w343:refnum<vi>)
        n158 = Not(x=w350) -> (.not. x?=w347:bool)
        n159 = Equal?(x=w349, y=T8."Run Time System" ("Application:Kind")) -> (x = y?=w346:bool)
        n160 = Or(x=w347, y=w346) -> (x .or. y?=w344:bool)
        n161 = Bundle By Name(cluster=w345, "Core.Current VI Reference"=w343, "Core.Close Panel on Exit?"=w344) -> (w352:T12)
        n162 = call <vilib>:"Add State(s) to Queue__jki_lib_state_machine.vi"("State(s) in (\"\")"=w354) -> ("States Out"=w353:string)  [unwired: 14 in]
      }
      frame "Error Handler" {
        # "Unhandled Error -- Display it"
        # "Handle any errors here.\nYou can also output any states to clean-up after errors occur"
        # "Clear error"
        n163 = call <vilib>:"General Error Handler.vi"("error in (no error)"=w356) -> ()  [unwired: 10 in, 5 out]
        n164 = call <vilib>:"Add State(s) to Queue__jki_lib_state_machine.vi"("State(s) in Front (\"\")"="/* Post Error States", "State(s) in (\"\")"=w360) -> ("States Out"=w359:string)  [unwired: 13 in]
      }
      frame "Exit" {
        # "Do not put any code in this frame.\n(No errors that occur here will be handled.)"
        n165 = call <vilib>:"Add State(s) to Queue__jki_lib_state_machine.vi"("State(s) in (\"\")"=w365) -> ("States Out"=w364:string)  [unwired: 14 in]
      }
      frame "---------- Data ----------" {
        # "Do not put any code in this frame.\n(It is a separator no-op. You can make a copy of this frame to create a new Data frame)"
        n166 = call <vilib>:"Add State(s) to Queue__jki_lib_state_machine.vi"("State(s) in (\"\")"=w369) -> ("States Out"=w368:string)  [unwired: 14 in]
      }
      frame "Data: Initialize" {
        w376 = T13 {"Config Strings"=[], "Config refs"=[]}  # Config
        w379 = FALSE  # Fire Continues Allowed
        w381 = u32 0  # Tik1
        w380 = u32 0  # Tik2
        w382 = FALSE  # Jet trigger
        w383 = 0.0  # Discharge timing offset
        w384 = 0.0  # Heater timing offset
        w385 = T14 {"Current VI Reference"=refnum, "Close Panel on Exit?"=FALSE}  # Core
        # "Data names and types of shift register data are defined by this bundle."
        # "Initialize the shift-register data, here.\n(data names are defined by what you wire into the bundle function)"
        n167 = control-ref of="value3::42"() -> (w378:refnum<vi>)
        n168 = control-ref of="value2::42"() -> (w377:refnum<vi>)
        n169 = control-ref of="value5::42"() -> (w371:refnum<vi>)
        n170 = control-ref of="value4::42"() -> (w372:refnum<vi>)
        n171 = control-ref of="value1::42"() -> (w370:refnum<vi>)
        n172 = Build Array(w378, w377, w372, w371, w370) -> (w374:refnum<vi>[])
        n173 = Bundle By Name(cluster=w376, "Config Strings"=string[] ["zpos for 0 above jet", "jet exit hpd for hexX0", "JetOnTime", "2BL probe 0 time pos", "focus on HPD"], "Config refs"=w374) -> (w373:T13)
        n174 = Bundle("Core"=w385, "Heater timing offset"=w384, "Discharge timing offset"=w383, "Jet trigger"=w382, "Tik1"=w381, "Tik2"=w380, "Fire Continues Allowed"=w379, "Config"=w373) -> (w387:T12)  [unwired: 1 in]
        n175 = call <vilib>:"Add State(s) to Queue__jki_lib_state_machine.vi"("State(s) in (\"\")"=w389) -> ("States Out"=w388:string)  [unwired: 14 in]
      }
      frame "Data: Cleanup" {
        # "Cleanup any data and references, here.\n(this is called automatically, by the Macro: Exit)"
        n176 = Unbundle By Name(w390) -> ("Core.Current VI Reference"=w393:refnum<vi>)
        n177 = Close Reference(reference=w393, error in (no error)=w392) -> (error out=w391:errorcluster)
        n178 = call <vilib>:"Add State(s) to Queue__jki_lib_state_machine.vi"("State(s) in (\"\")"=w395) -> ("States Out"=w394:string)  [unwired: 14 in]
      }
      frame "---------- UI ----------" {
        # "Do not put any code in this frame.\n(It is a separator no-op. You can make a copy of this frame to create a new UI frame)"
        n179 = call <vilib>:"Add State(s) to Queue__jki_lib_state_machine.vi"("State(s) in (\"\")"=w399) -> ("States Out"=w398:string)  [unwired: 14 in]
      }
      frame "UI: Initialize" {
        # "Initialize the User Interface, here.\n(this is called automatically, by the Macro: Init)"
        n180 = call <userlib>:"Fit VI window to Largest Dec__ogtk.vi"() -> ()  [unwired: 6 in, 2 out]
        n181 = call <vilib>:"Add State(s) to Queue__jki_lib_state_machine.vi"("State(s) in (\"\")"=w403) -> ("States Out"=w402:string)  [unwired: 14 in]
      }
      frame "Action: Config File Read" {
        n182 = disable-structure shown="Enabled" {
          disable-tunnel: w406 -> [w413 w435]
          disable-tunnel: [w412 w435] -> w405
          disable-tunnel: w404 -> [w411 _]
          frame Disabled {
            n183 = Unbundle By Name(w411) -> ("Config.Config Strings"=w410:string[], "Config.Config refs"=w409:refnum<vi>[])
            n184 = call <vilib>:"Open Config Data.vi"("error in (no error)"=w413, "create file if necessary (T)"=FALSE, "configuration file path"="configuration file path") -> ("error out"=w414:errorcluster, "refnum"=w418:T11)  [unwired: 6 in, 1 out]
            n185 = for {
              shift-right: [w428] -> w417
              shift-left: w418 -> [w429]
              shift-right: [w422] -> w416
              shift-left: w414 -> [w427]
              tunnel: w410 -> [w426] mode=indexing
              tunnel: w409 -> [w421] mode=indexing
              n186 = call-poly <vilib>:"Read Key.vi"("section"="BCC", "error in (no error)"=w427, "key"=w426, "refnum"=w429) -> ("error out"=w423:errorcluster, "value"=w424:dbl, "found?"=w420:bool, "refnum out"=w428:T11)  [unwired: 4 in]
              n187 = case shown="True" w420 {
                tunnel: w424 -> [_ w434]
                tunnel: w423 -> [w430 w433]
                tunnel: [w430 w432] -> w422
                tunnel: w421 -> [_ w431]
                frame False {
                }
                frame True {
                  n188 = property class="DigNum (strict)"(reference=w431, error in=w433, "Value"=w434) -> (error out=w432:errorcluster)  [unwired: 1 out]
                }
              }
            }
            n189 = call <vilib>:"Close Config Data.vi"("error in (no error)"=w416, "refnum"=w417) -> ("error out"=w412:errorcluster)  [unwired: 8 in, 1 out]
          }
          frame Enabled {
          }
        }
        n190 = call <vilib>:"Add State(s) to Queue__jki_lib_state_machine.vi"("State(s) in (\"\")"=w408) -> ("States Out"=w407:string)  [unwired: 14 in]
      }
      frame "Action: Config File Save" {
        n191 = disable-structure shown="Enabled" {
          disable-tunnel: w438 -> [w445 _]
          disable-tunnel: w437 -> [w443 w460]
          disable-tunnel: [w442 w460] -> w436
          frame Disabled {
            n192 = Unbundle By Name(w445) -> ("Config.Config Strings"=w444:string[], "Config.Config refs"=w441:refnum<vi>[])
            n193 = local read "configuration file path"() -> (w450:path)
            n194 = call <vilib>:"Open Config Data.vi"("create file if necessary (T)"=TRUE, "configuration file path"=w450) -> ("refnum"=w447:T11)  [unwired: 7 in, 2 out]
            n195 = for {
              tunnel: [w459] -> w449
              tunnel: w444 -> [w456] mode=indexing
              shift-right: [w458] -> w448
              shift-left: w447 -> [w457]
              tunnel: w443 -> [w452]
              tunnel: w441 -> [w451] mode=indexing
              n196 = property class="DigNum (strict)"(reference=w451, error in=w452) -> (error out=w453:errorcluster, "Value"=w454:dbl)  [unwired: 1 out]
              n197 = call-poly <vilib>:"Write Key.vi"("section"="BCC", "error in (no error)"=w453, "value"=w454, "key"=w456, "refnum"=w457) -> ("error out"=w459:errorcluster, "refnum out"=w458:T11)  [unwired: 4 in, 1 out]
            }
            n198 = call <vilib>:"Close Config Data.vi"("error in (no error)"=w449, "refnum"=w448) -> ("error out"=w442:errorcluster)  [unwired: 8 in, 1 out]
          }
          frame Enabled {
          }
        }
        n199 = call <vilib>:"Add State(s) to Queue__jki_lib_state_machine.vi"("State(s) in (\"\")"=w440) -> ("States Out"=w439:string)  [unwired: 14 in]
      }
      frame "UI: Cursor Set" {
        # "Argument"
        # "Set and Unset Cursor Busy.\n(Usage: \"UI: Cursor Set >> Busy|Idle\")"
        n200 = case shown="\"Idle\", Default" w461 {
          tunnel: w463 -> [w468 w470]
          tunnel: [w467 w469] -> w462
          frame "Idle", Default {
            n201 = call <vilib>:"Unset Busy.vi"("error in (no error)"=w468) -> ("error out"=w467:errorcluster)  [unwired: 10 in]
          }
          frame "Busy" {
            n202 = call <vilib>:"Set Busy.vi"("error in (no error)"=w470) -> ("error out"=w469:errorcluster)  [unwired: 9 in, 1 out]
          }
        }
        n203 = call <vilib>:"Add State(s) to Queue__jki_lib_state_machine.vi"("State(s) in (\"\")"=w466) -> ("States Out"=w465:string)  [unwired: 14 in]
      }
      frame "UI: Front Panel State" {
        # "Argument"
        # "Set Front Panel Open or Closed\n(Usage: \"UI: Front Panel State >> Open|Close\")"
        n204 = Unbundle By Name(w473) -> ("Core.Current VI Reference"=w472:refnum<vi>)
        n205 = case shown="\"Close\"" w471 {
          tunnel: w475 -> [w481 w494]
          tunnel: [w483 w495] -> w474
          tunnel: w472 -> [w482 w492]
          frame "Open", Default {
            n206 = property class="VI"(reference=w482, error in=w481) -> (reference out=w479:refnum<vi>, error out=w480:errorcluster, "Front Panel.Open"=w478:bool)
            n207 = case shown="False" w478 {
              tunnel: [w486 w489] -> w483
              tunnel: w480 -> [w485 w489]
              tunnel: w479 -> [w484 _]
              frame False {
                n208 = invoke class="VI" method="FP.Open"(reference=w484, error in=w485, "Activate"=TRUE, "State"=T9."Standard") -> (error out=w486:errorcluster)  [unwired: 1 in, 4 out]
              }
              frame True {
              }
            }
          }
          frame "Close" {
            n209 = property class="VI"(reference=w492, error in=w494) -> (reference out=w491:refnum<vi>, error out=w493:errorcluster, "Front Panel.Open"=w490:bool)
            n210 = case shown="True" w490 {
              tunnel: [w496 w499] -> w495
              tunnel: w493 -> [w496 w498]
              tunnel: w491 -> [_ w497]
              frame False {
              }
              frame True {
                n211 = invoke class="VI" method="FP.Close"(reference=w497, error in=w498) -> (error out=w499:errorcluster)  [unwired: 1 in, 2 out]
              }
            }
          }
        }
        n212 = call <vilib>:"Add State(s) to Queue__jki_lib_state_machine.vi"("State(s) in (\"\")"=w477) -> ("States Out"=w476:string)  [unwired: 14 in]
      }
      frame "---------- Macro ----------" {
        # "Do not put any code in this frame.\n(It is a separator no-op. You can make a copy of this frame to create a new Macro frame)"
        n213 = call <vilib>:"Add State(s) to Queue__jki_lib_state_machine.vi"("State(s) in (\"\")"=w503) -> ("States Out"=w502:string)  [unwired: 14 in]
      }
      frame "Macro: Initialize" {
        w504 = "Data: Initialize\nInitialize Core Data\nUI: Initialize\nUI: Front Panel State >> Open\nCheck if Fire continues allowed\nInitilize Fire Continues\nAction: Config File Read\nInit:MegattenuatorStage"  # Data: Initialize Initialize Core Data UI: Initialize UI: Front Panel State >> Open Check if Fire continues allowed Initilize Fire Continues Action: Config File Read Init:MegattenuatorStage
        # "Initialization Macro\n(This is called once, when the VI starts)"
        n214 = call <vilib>:"Add State(s) to Queue__jki_lib_state_machine.vi"("State(s) in Front (\"\")"=w504, "State(s) in (\"\")"=w508) -> ("States Out"=w507:string)  [unwired: 13 in]
      }
      frame "Macro: Exit" {
        # "Exit Macro\n(This is called once, when the VI exits)"
        n215 = Unbundle By Name(w518) -> ("Core.Close Panel on Exit?"=w517:bool)
        n216 = Release Queue(queue=w510, force destroy? (F)=TRUE) -> (error out=w509:errorcluster)  [unwired: 1 in, 2 out]
        n217 = call <vilib>:"Clear Errors.vi"("error in (no error)"=w509) -> ()  [unwired: 5 in, 2 out]
        n218 = Select(t="UI: Front Panel State >> Close", s=w517, f="") -> (s? t:f=w514:string)
        n219 = call <vilib>:"Add State(s) to Queue__jki_lib_state_machine.vi"("State(s) in (\"\")"=w514, "State(s) at Back (\"\")"="Data: Cleanup\nExit") -> ("States Out"=w512:string)  [unwired: 13 in]
        n220 = call <vilib>:"Add State(s) to Queue__jki_lib_state_machine.vi"("State(s) in Front (\"\")"=w512, "State(s) in (\"\")"=w521) -> ("States Out"=w520:string)  [unwired: 13 in]
      }
      frame "---------- New Category ----------" {
        # "Template Separator\n(You can make a copy of, or modify, this frame)"
        n221 = call <vilib>:"Add State(s) to Queue__jki_lib_state_machine.vi"("State(s) in (\"\")"=w525) -> ("States Out"=w524:string)  [unwired: 14 in]
      }
      frame "Check Megattenuator Stage Status" {
        # "Template Separator\n(You can make a copy of, or modify, this frame)"
        n222 = Tick Count (ms)() -> (millisecond timer value=w526:u32)
        n223 = while {
          tunnel: w527 -> [w539]
          tunnel: w526 -> [w537]
          stop <- w532 stop-if-true
          n224 = flat-sequence {
            tunnel: [w543] -> w540
            frame #0 {
              n225 = Wait (ms)(milliseconds to wait=u32 250) -> ()  [unwired: 1 out]
            }
            frame #1 {
              n226 = property on="Position.Ch1::44" class="DigNum (strict)"() -> ("Value"=w544:dbl)  [unwired: 2 in, 2 out]
              n227 = case shown="149..151" w544 {
                tunnel: ["IN" "Unknown/Moving" "OUT"] -> w543
                frame 0, 1 {
                  n228 = property on="MoveStage" class="Bool (strict)"("Value"=TRUE) -> ()  [unwired: 2 in, 2 out]
                }
                frame 2, Default {
                }
                frame 149..151 {
                  n229 = property on="MoveStage" class="Bool (strict)"("Value"=FALSE) -> ()  [unwired: 2 in, 2 out]
                }
              }
            }
          }
          n230 = Tick Count (ms)() -> (millisecond timer value=w538:u32)
          n231 = Wait (ms)(milliseconds to wait=u32 750) -> ()  [unwired: 1 out]
          n232 = Subtract(x=w538, y=w537) -> (x-y=w536:u32)
          n233 = Greater?(x=w536, y=u32 30000) -> (0:w533:bool)
          n234 = Equal?(x=w540, y=w539) -> (x = y?=w534:bool)
          n235 = property on="CurrentStatus" class="Str"("Value"=w540) -> ()  [unwired: 2 in, 2 out]
          n236 = Or(x=w534, y=w533) -> (x .or. y?=w532:bool)
        }
        n237 = call <vilib>:"Add State(s) to Queue__jki_lib_state_machine.vi"("State(s) in (\"\")"=w531) -> ("States Out"=w530:string)  [unwired: 14 in]
      }
      frame "Init:MegattenuatorStage" {
        # "Template Separator\n(You can make a copy of, or modify, this frame)"
        n238 = flat-sequence {
          frame #0 {
            n239 = call <vilib>:"Set Busy.vi"("disable click? (T)"=TRUE, "cursor ID"=refnum<k1> refnum) -> ()  [unwired: 8 in, 2 out]
          }
          frame #1 {
            n240 = while {
              tunnel: [w565] -> w557
              i -> [w560]
              stop <- w561 stop-if-true
              n241 = property on="Position.Ch1::44" class="DigNum (strict)"() -> ("Value"=w565:dbl)  [unwired: 2 in, 2 out]
              n242 = Equal?(x=50, y=w560) -> (x = y?=w558:bool)
              n243 = Not Equal?(x=w565, y=0.0) -> (x != y?=w562:bool)
              n244 = Wait (ms)(milliseconds to wait=u32 100) -> ()  [unwired: 1 out]
              n245 = Or(x=w562, y=w558) -> (x .or. y?=w561:bool)
            }
            n246 = case shown="0, 1" w557 {
              tunnel: ["IN" "Unknown" "OUT"] -> w556
              frame 0, 1 {
                n247 = property on="MoveStage" class="Bool (strict)"("Value"=TRUE) -> ()  [unwired: 2 in, 2 out]
              }
              frame 2, Default {
                n248 = property on="MoveStage" class="Bool (strict)"("DisabledEnum"=T7."Disabled" ("Disabled")) -> ()  [unwired: 2 in, 2 out]
              }
              frame 149..151 {
                n249 = property on="MoveStage" class="Bool (strict)"("Value"=FALSE) -> ()  [unwired: 2 in, 2 out]
              }
            }
            n250 = property on="CurrentStatus" class="Str"("Value"=w556) -> ()  [unwired: 2 in, 2 out]
          }
          frame #2 {
            n251 = call <vilib>:"Unset Busy.vi"() -> ()  [unwired: 11 in, 1 out]
          }
        }
        n252 = call <vilib>:"Add State(s) to Queue__jki_lib_state_machine.vi"("State(s) in (\"\")"=w553) -> ("States Out"=w552:string)  [unwired: 14 in]
      }
      frame "CheckTimeFire" {
        # "Your code here.\n(You can make a copy of, or modify, this frame)"
        n253 = Unbundle By Name(w578) -> ("Tik1"=w583:u32)
        n254 = Tick Count (ms)() -> (millisecond timer value=w585:u32)
        n255 = Unbundle By Name(w578) -> ("Fire Continues Allowed"=w575:bool)
        n256 = Reciprocal(x="Rate (Hz)") -> (1/x=w574:dbl)
        n257 = Subtract(x=w585, y=w583) -> (x-y=w586:u32)
        n258 = Multiply(x=1000.0, y=w574) -> (x*y=w573:dbl)
        n259 = Greater?(x=w586, y=w573) -> (0:w581:bool)
        n260 = And(x=w581, y="value0::22") -> (x .and. y?=w577:bool)
        n261 = And(x=w575, y=w577) -> (x .and. y?=w576:bool)
        n262 = case shown="True" w576 {
          tunnel: w585 -> [_ w593]
          tunnel: [w591 w593] -> w584
          tunnel: w583 -> [w591 _]
          tunnel: [_ "Action: Fire" ("State(s) in Front (\"\")")] -> w580
          frame False {
          }
          frame True {
          }
        }
        n263 = Bundle By Name(cluster=w578, "Tik1"=w584) -> (w587:T12)
        n264 = call <vilib>:"Add State(s) to Queue__jki_lib_state_machine.vi"("State(s) in Front (\"\")"=w580, "State(s) in (\"\")"=w590) -> ("States Out"=w589:string)  [unwired: 13 in]
        "Fire continues Indicator" <- "value0::22"
      }
      frame "Initilize Fire Continues" {
        # "Your code here.\n(You can make a copy of, or modify, this frame)"
        n265 = Unbundle By Name(w597) -> ("Fire Continues Allowed"=w596:bool)
        n266 = property on="value0::22" class="Bool (strict)"(error in=w599, "Visible"=w596) -> (error out=w598:errorcluster)  [unwired: 1 in, 1 out]
        n267 = Not(x=w596) -> (.not. x?=w594:bool)
        n268 = property on="Fire continues Indicator" class="Bool (strict)"(error in=w598, "Visible"=w594) -> (error out=w595:errorcluster)  [unwired: 1 in, 1 out]
        n269 = call <vilib>:"Add State(s) to Queue__jki_lib_state_machine.vi"("State(s) in (\"\")"=w601) -> ("States Out"=w600:string)  [unwired: 14 in]
      }
      frame "Check if Fire continues allowed" {
        # "Check if it is allowed computer"
        # "Your code here.\n(You can make a copy of, or modify, this frame)"
        n270 = String To IP() -> (0:w609:u32)  [unwired: 1 in]
        n271 = IP To String(1:TRUE ("dot notation? (F)"), 2:w609) -> (0:w610:string)
        n272 = Equal?(x=w610, y="192.168.14.2") -> (x = y?=w604:bool)
        n273 = Not(x=w604) -> (.not. x?=w605:bool)
        n274 = Bundle By Name(cluster=w607, "Fire Continues Allowed"=w604) -> (w606:T12)
        n275 = property on="Allow Fire Continues" class="Bool (strict)"(error in=w603, "Visible"=w605) -> (error out=w602:errorcluster)  [unwired: 1 in, 1 out]
        n276 = call <vilib>:"Add State(s) to Queue__jki_lib_state_machine.vi"("State(s) in (\"\")"=w613) -> ("States Out"=w612:string)  [unwired: 14 in]
      }
      frame "CheckTime2" {
        # "Your code here.\n(You can make a copy of, or modify, this frame)"
        n277 = Unbundle By Name(w622) -> ("Tik2"=w615:u32)
        n278 = Tick Count (ms)() -> (millisecond timer value=w617:u32)
        n279 = Subtract(x=w617, y=w615) -> (x-y=w620:u32)
        n280 = Greater?(x=w620, y=5000) -> (0:w618:bool)
        n281 = case shown="True" w618 {
          tunnel: w617 -> [_ w628]
          tunnel: [w626 w628] -> w616
          tunnel: w615 -> [w626 _]
          tunnel: [_ "Action: update expt vars\nAction: save screenshot"] -> w614
          frame False {
          }
          frame True {
          }
        }
        n282 = Bundle By Name(cluster=w622, "Tik2"=w616) -> (w621:T12)
        n283 = call <vilib>:"Add State(s) to Queue__jki_lib_state_machine.vi"("State(s) in Front (\"\")"=w614, "State(s) in (\"\")"=w625) -> ("States Out"=w624:string)  [unwired: 13 in]
      }
      frame "Action: Fire" {
        n284 = property on="fire::10" class="Str"(error in=w630, "Val(Sgnl)"="fire>>force" ("Value (Signaling)")) -> (error out=w629:errorcluster)  [unwired: 1 in, 1 out]
        n285 = call <vilib>:"Add State(s) to Queue__jki_lib_state_machine.vi"("State(s) in (\"\")"=w634) -> ("States Out"=w633:string)  [unwired: 14 in]
      }
      frame "Action: MoveCap" {
        n286 = local read "ypos::1"() -> (w649:dbl)
        n287 = case shown="\"In\"" w645 {
          tunnel: [25.0 ("Value (Signaling)") 0.0 ("Value (Signaling)")] -> w644
          tunnel: [-20.0 ("x") 20.0 ("x")] -> w643
          frame "In" {
          }
          frame "Out", Default {
          }
        }
        n288 = Add(x=w643, y=w649) -> (x+y=w648:dbl)
        n289 = property on="ypos::1" class="DigNum (strict)"(error in=w647, "Val(Sgnl)"=w648) -> (error out=w646:errorcluster)  [unwired: 1 in, 1 out]
        n290 = property on="EnableMotor::6" class="Bool (strict)"("Val(Sgnl)"=TRUE ("Value (Signaling)")) -> (error out=w641:errorcluster)  [unwired: 2 in, 1 out]
        n291 = call <userlib>:"Wait (ms)__ogtk.vi"("error in (no error)"=w641, "milliseconds to wait"=u32 1000) -> ("error out"=w640:errorcluster)  [unwired: 8 in, 1 out]
        n292 = property on="position::4" class="DigNum (strict)"(error in=w640, "Val(Sgnl)"=w644) -> (error out=w637:errorcluster)  [unwired: 1 in, 1 out]
        n293 = call <userlib>:"Wait (ms)__ogtk.vi"("error in (no error)"=w637, "milliseconds to wait"=u32 6000) -> ("error out"=w635:errorcluster)  [unwired: 8 in, 1 out]
        n294 = property on="EnableMotor::6" class="Bool (strict)"(error in=w635, "Val(Sgnl)"=FALSE ("Value (Signaling)")) -> ()  [unwired: 1 in, 2 out]
        n295 = call <vilib>:"Add State(s) to Queue__jki_lib_state_machine.vi"("State(s) in (\"\")"=w652) -> ("States Out"=w651:string)  [unwired: 14 in]
      }
      frame "Action: update expt vars" {
        # "Your code here.\n(You can make a copy of, or modify, this frame)"
        n296 = call <vilib>:"Add State(s) to Queue__jki_lib_state_machine.vi"("State(s) in (\"\")"=w660) -> ("States Out"=w659:string)  [unwired: 14 in]
      }
      frame "Action: SendScanParameters" {
        # "Your code here.\n(You can make a copy of, or modify, this frame)"
        n297 = call "BELLA PW scan mode shot control shutter.vi"("ScanShotControl"="value0::43") -> ("error out"=w663:errorcluster)  [unwired: 10 in]
        n298 = call "Jet in scan on or off.vi"("error in (no error)"=w663, "gas jet on time"="value4::42", "GasJetOn"="value1::43") -> ()  [unwired: 8 in, 1 out]
        n299 = call <vilib>:"Add State(s) to Queue__jki_lib_state_machine.vi"("State(s) in (\"\")"=w668) -> ("States Out"=w667:string)  [unwired: 14 in]
      }
      frame "Action: save screenshot" {
        # "Your code here.\n(You can make a copy of, or modify, this frame)"
        n300 = case shown="True" "Save screenshots" {
          frame False {
          }
          frame True {
            n301 = invoke class="VI" method="FP.Get Image"() -> ("image data"=w676:T10)  [unwired: 6 in, 5 out]
            n302 = call <vilib>:"Write PNG File.vi"("image data"=w676, "path to PNG file"=path "N:/data/ECS dumps/Logmaker Screenshot/frontpanel.png" ("report file path")) -> ("error out"=→"error out":errorcluster)  [unwired: 8 in, 1 out]
          }
        }
        n303 = call <vilib>:"Add State(s) to Queue__jki_lib_state_machine.vi"("State(s) in (\"\")"=w673) -> ("States Out"=w672:string)  [unwired: 14 in]
      }
    }
  }
  n304 = disable-structure shown="Disabled" {
    frame Disabled {
      n305 = call "DefaultValue_Variable_MC.vi"() -> ()  [unwired: 4 in]
    }
    frame Enabled {
    }
  }
  n306 = disable-structure shown="Disabled" {
    frame Disabled {
    }
    frame Enabled {
    }
  }
  n307 = disable-structure shown="Disabled" {
    frame Disabled {
    }
    frame Enabled {
    }
  }
  n308 = disable-structure shown="Disabled" {
    frame Disabled {
    }
    frame Enabled {
    }
  }
  "CurrentStatus" <- ""
